vi "DepthProfiling_3D_Core.vi"(5 "BioMAP file path":path=path "", 7 "Params.":variant, 8 "error in (no error)":errorcluster, 9 "Dynamic Params queue":refnum<queue>, 10 "Quit_UserEvent":refnum<user-event>, 11 "ControlQueueRef":variant) -> (0 "error out":errorcluster, 2 "Output":variant)   [LabVIEW 2013]
uses:
  Apps_static/ScanParams_SingleLine.ctl
  ProcessMethods/Binning/BinType.ctl
  Files/BinaryHeader.ctl
  ControlDef/QueueRefs.ctl
  ControlDef/LaserCtrl_Method.ctl
  ControlDef/States-AToF.ctl
  <instrlib>/AnalogDiscSDKLv/VIs/DWF_CtrlQueue.ctl
  <instrlib>/AnalogDiscSDKLv/VIs/DWF_State.ctl
  <instrlib>/ESP300/Public/Data/ESP300_State.ctl
  <instrlib>/DG535/Command/DG535_States.ctl
  Hardware/BNC(QuantumComposers)/BNC_States.ctl
  Hardware/FemtoLaser(Legacy)/Laser_Status.ctl
  Hardware/DAQmx(Legacy)/DAQmx_Status.ctl
  ControlDef/Signal.ctl
  ProcessMethods/SignalAverager/ProcessStates.ctl
  Files/WriterState.ctl
  Files/Signal_Segment.ctl
  ControlDef/ProcessingMode.ctl
  Hardware/EPM2000(Legacy)/EPM2K_Status.ctl
  <instrlib>/AnalogDiscSDKLv/VIs/DWF_Signal.ctl
  ControlDef/SampleRateSelector.ctl
  ImagingMS/DirectImaging_State.ctl
  ImagingMS/Imaging_Params.ctl
  ProcessMethods/BioMapConversion/BioMAPWriterCoreParams.ctl
  <vilib>/Utility/error.llb/DialogType.ctl
  <vilib>/Utility/miscctls.llb/LVRowAndColumnTypeDef.ctl
  <vilib>/picture/picture.llb/imagedata.ctl
  <vilib>/Analysis/baseanly.llb/Mean (DBL).vi
  UI/Autoscale_Y_Single.vi
  <userlib>/_OpenG.lib/comparison/comparison.llb/I32 Changed__ogtk.vi
  ProcessMethods/Binning/SpectrumBinning.vi
  <vilib>/regexp/Match Regular Expression.xnode
  <instrlib>/ESP300/ESP300.lvlib
  <instrlib>/DG535/SRS_DG535_Lib.lvlib
  <userlib>/Utility/ErrorLog_lib.lvlib
  <instrlib>/AnalogDiscSDKLv/AnalogDiscSDKLv.lvlib
  <vilib>/Analysis/NI_AALBase.lvlib
panel:
  out "m/z":dbl=11.0
  in  "Linear/Log":bool
  in  "Integration Width (±Da)":dbl=0.5
  in  "m/z (Da)":dbl=11.0
  in  "BinType":T1=enum."ByMass"
  in  "BinWidth":dbl=0.2 min=0.001
  in  "#Layers":i32=1 caption="LayerAverage#" min=1 max=2000 step=1
  in  "Shot#":i32=1 caption="nth of Shot" min=1 max=65535 step=1
  in  "X--":bool
  in  "X++":bool
  in  "Fullscale X":bool
  in  "Fullscale Y":bool
  in  "Y--":bool
  in  "Y++":bool
  out "Depth Profile":dbl[](graph)
  out "Spectra":cluster{"Array":dbl[], dbl[]}(graph)
  in  "MaxiMass":dbl=300.0 format="%#_13g"
  in  "EnableBinning":bool
  out "Information":string
  in  "AutoScaleZ":bool
  in  "SaveMiddleFile":bool
  in  "Color Scheme":T2(ring)=enum."Rainbow"
  out "#SOL":i32
  out "#EOL":i32
  out "remaining lines":i32
  out "State":T3(ring)
  out "Line#":i32
  in  "Cancel":bool
  in  "Close/Quit":bool
  in  "Peaks of Interest":string[][](table)=[["300", "300"], ["68", ".45"], ["92", ".45"], ["114", ".45"]]
  in  "conv. coeff.":sgl=6553.0
  out "# average":i32
  in  "Start":bool
  out "ImagePreview":dbl[][](graph)
  in  "PeakOI #":i32
  out "MS (Raw)":cluster{"m/z_Array":dbl[], sgl[]}(graph)
  out "Iteration":i32
  out "Export File Path":path caption="Filename"
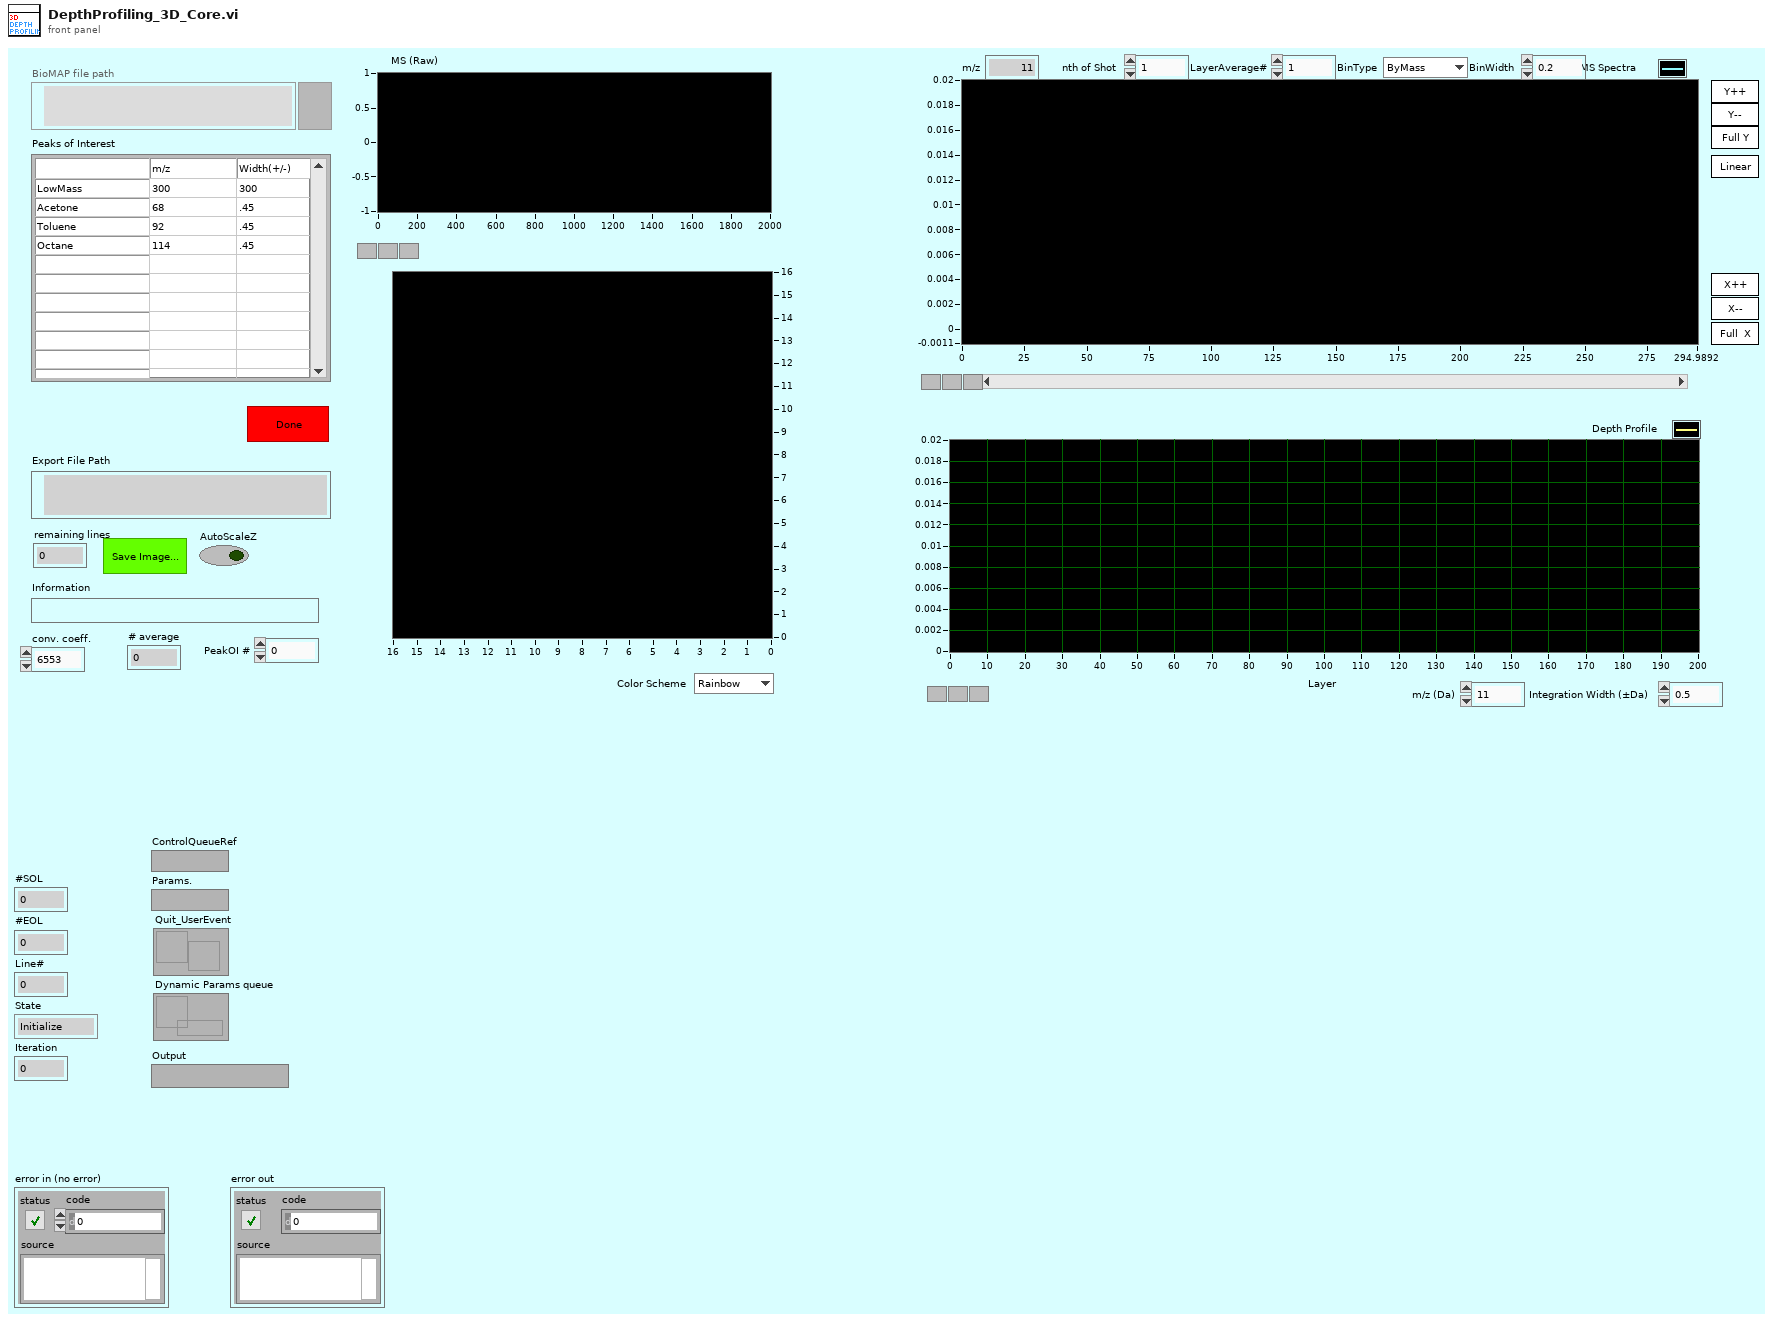
[diagram p1: front panel]
types:
  T1 = typedef "BinType.ctl" = enum16{"ByTime", "ByScreen", "ByMass", "ToUnitMass"}
  T2 = enum16{"Greyscale", "Rainbow", "Jet", "Rainbow_Wh", "Banded", "Seis", "InvertSeis", "Jaisnd", "TBD1"}
  T3 = enum16{"Initialize", "Open", "PrepScanParams", "WaitData", "Flush", "ScanResult", "CheckEndCondition", "Close", "Quit", "Refresh_Image", "Refresh_Profile", "Refresh_Spectra", "Refresh_RawSpectrum", "SaveMiddleFile", "Save_Image", "SetPeakOI"}
  T4 = cluster{"image path":path, "file refnum":refnum<file>}
  T5 = enum8{"Enabled", "Disabled", "Disabled and Grayed Out"}
  T6 = typedef "QueueRefs.ctl" = cluster{"LaserCtrlMethod":T7, "Apps":refnum<queue>, "MainDAQCoreQueue":refnum<queue>, "Micos":refnum<queue>, "ESP300":refnum<queue>, "SMC100":refnum<queue>, "SRS DG535":refnum<queue>, "BNC":refnum<queue>, "SDG_ii":refnum<queue>, "NI-USB_DAQmx":refnum<queue>, "ProcCore_CtrlQueue":refnum<queue>, "WriterCtrl":refnum<queue>, "WriterSIG":refnum<queue>, "Feedback":refnum<queue>, "EPM2000":refnum<queue>, "InfoRef":refnum<vi>, "AppsLock":T8, "ProcCore_SignalQueue":refnum<queue>}
  T7 = typedef "LaserCtrl_Method.ctl" = enum16{"SRS_DG535", "BNC", "SDG_II"}
  T8 = typedef "Semaphore RefNum" = refnum<k1>
  T9 = typedef "ProcessStates.ctl" = enum16{"Initialize", "Normal", "Display", "Write2Buffer", "CalcMzArray", "StartSave", "StopSave", "ConfigChanged", "EndOfLine", "SetFilterParams", "SetGraphsEnable", "SetAcquisitionParams", "ChangeDisplayIncrement", "ChangeRepRate", "SetWriterRef", "Quit", "StartOfLine"}
  T10 = cluster{"Average":i32, "X (Img)":i32, "Y (Img)":i32, "Spectra":sgl[], "Depth":i32, "TickCount":dbl}
  T11 = typedef "BioMAPWriterCoreParams.ctl" = cluster{"File Header":T12, "mzCali.":dbl[], "m/z_Array":dbl[], "SampleRate":T13, "TrigDelay":dbl, "file refnum":refnum<file>, "file path":path, "PeakOI":cluster{"m/z":dbl, "Width(+/-)":dbl}[], "Binning":cluster{"Enable":bool, "BinType":T1, "BinWidth":dbl, "Maximum":dbl, "Minimum":dbl}}
  T12 = typedef "BinaryHeader.ctl" = cluster{"Start Position":dbl[], "StepWidth":dbl[], "Dimension":i32[], "SpecLength":i32}
  T13 = typedef "SampleRateSelector.ctl" = dbl
  T14 = typedef "Imaging_Params.ctl" = cluster{"File Header":T12, "ScanSpeed":dbl, "HighSpeed":dbl, "SampleRate":T13, "Rep.Rate (Hz)":dbl, "TrigDelay":dbl, "mzCali":dbl[], "KeepStill(ms)":u32, "SaveRaw":bool}
  T15 = typedef "DirectImaging_State.ctl" = cluster{"State":enum16{"Initialize", "Open", "PrepScanParams", "WaitData", "Flush", "ScanResult", "CheckEndCondition", "Close", "Quit", "Refresh_Image", "Refresh_Profile", "Refresh_Spectra", "Refresh_RawSpectrum", "SaveMiddleFile", "Save_Image", "SetPeakOI"}, "Para.":variant}
  T16 = cluster{"Save?":bool, "File Header":T12, "Scan#":i32, "ControlRefs":T6, "HighSpeed":dbl, "ScanSpeed":dbl, "SampleRate":T13, "mzCali.":dbl[], "TrigDelay":dbl, "InfoBarRef.":refnum<vi>, "mzArray":dbl[], "SaveRaw":bool, "RepRate":dbl, "Z_Counter":i32}
  T17 = typedef "LVRowAndColumnTypeDef.ctl" = cluster{"Row":i32, "Column":i32}
  T18 = typedef "DialogType.ctl" = u16
  T19 = typedef "LVPoint32TypeDef.ctl" = cluster{"Horizontal":i32, "Vertical":i32}
  T20 = typedef "LVRectTypeDef.ctl" = cluster{"Left":i16, "Top":i16, "Right":i16, "Bottom":i16}
  T21 = enum16{"open", "replace", "create", "open or create", "replace or create", "replace or create with confirmation"}
  T22 = cluster{"queue out":refnum<queue>, "queue out":refnum<queue>}
  T23 = typedef "Signal.ctl" = cluster{"Command":T9, "Params":variant}
  T24 = typedef "Signal_Segment.ctl" = cluster{"SampleRate":dbl, "TrigDelay":dbl, "SpecLength":dbl, "DAQ_Range":dbl, "Average#":i32, "Position":dbl[], "Spectrum":sgl[], "Calibr.":dbl[], "Pressure":dbl, "Desp_LaserEnergy":dbl, "PI_LaserEnergy":dbl, "Voltages Table":sgl[][], "ProcMode":T25, "Threshold":dbl, "Comment":string, "TickCount":dbl, "Time Stamp":timestamp}
  T25 = typedef "ProcessingMode.ctl" = enum16{"None", "Drop by Threshold", "TDC Simulate", "SetFilter"}
  T26 = typedef "ScanParams_SingleLine.ctl" = cluster{"Line Start":dbl[], "Line End":dbl[], "HighSpeed":dbl, "ScanSpeed":dbl, "KeepStill(ms)":u32, "InstruParams":dbl[]}
  T27 = typedef "imagedata.ctl" = cluster{"image type":i32, "image depth":i32, "image":u8[], "mask":u8[], "colors":u32[], "Rectangle":cluster{"left":i16, "top":i16, "right":i16, "bottom":i16}}
  T28 = cluster{"Rows Per Strip":i32, "Photometric":i32, "Compression Type":i32}
  T29 = cluster{"Average":i32, "X (Img)":i32, "Y (Img)":i32, "Spectra":sgl[], "Depth":i32, "TickCount":dbl}[]
  T30 = typedef "IMAQ Image.ctl" = refnum<image>
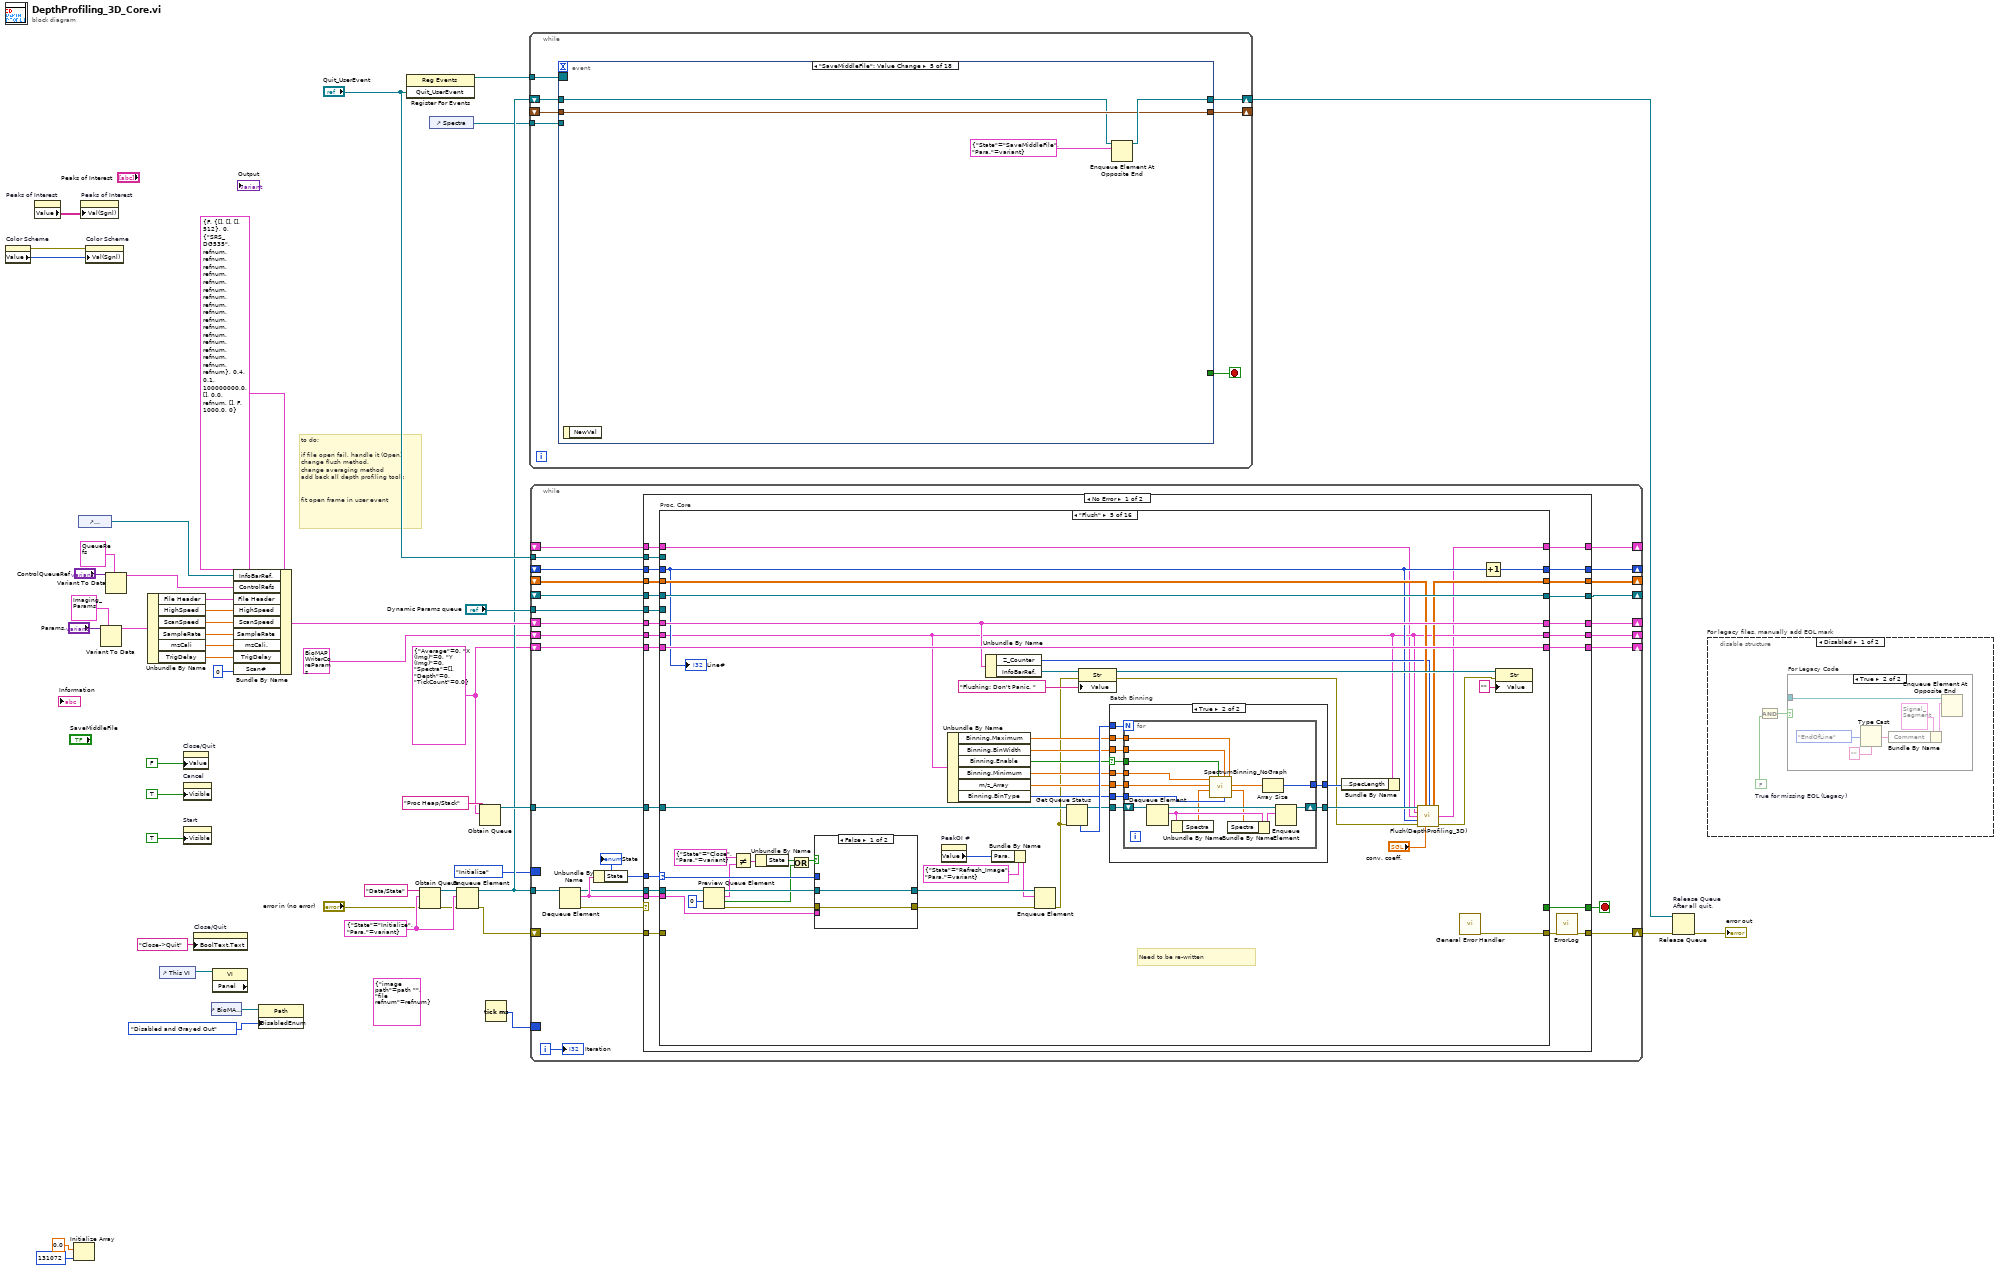
[diagram p0: block diagram]
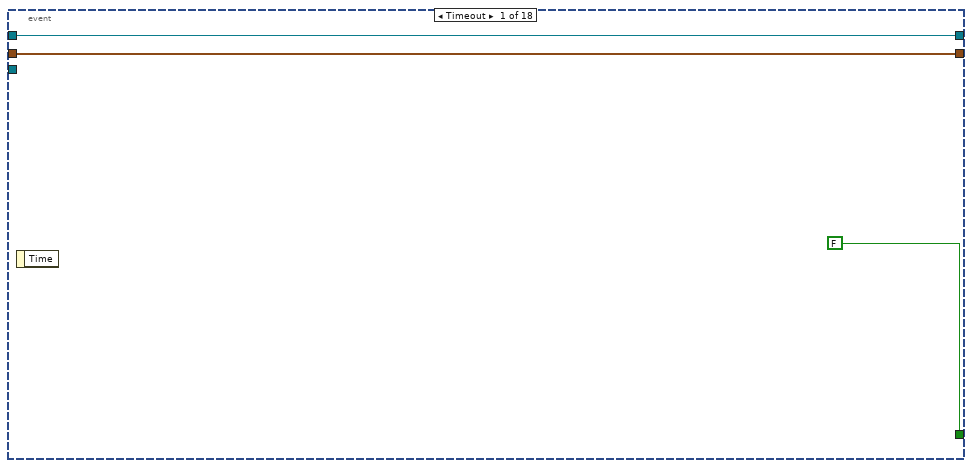
[diagram p4: hidden frame]
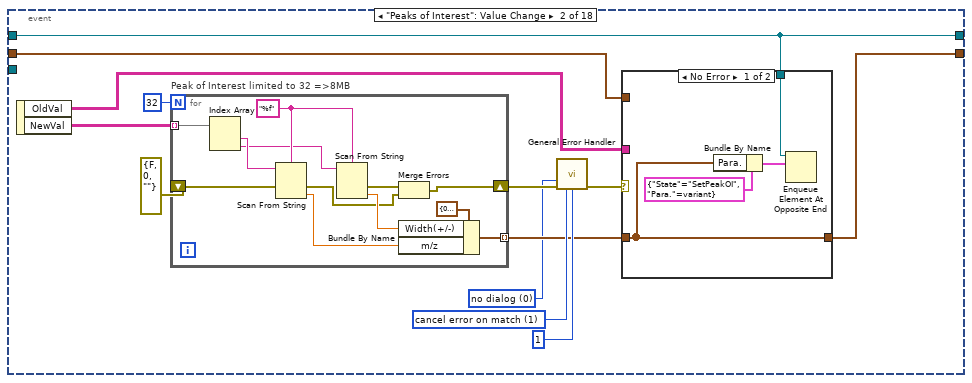
[diagram p5: hidden frame]
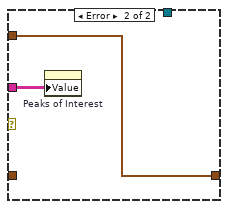
[diagram p6: hidden frame]
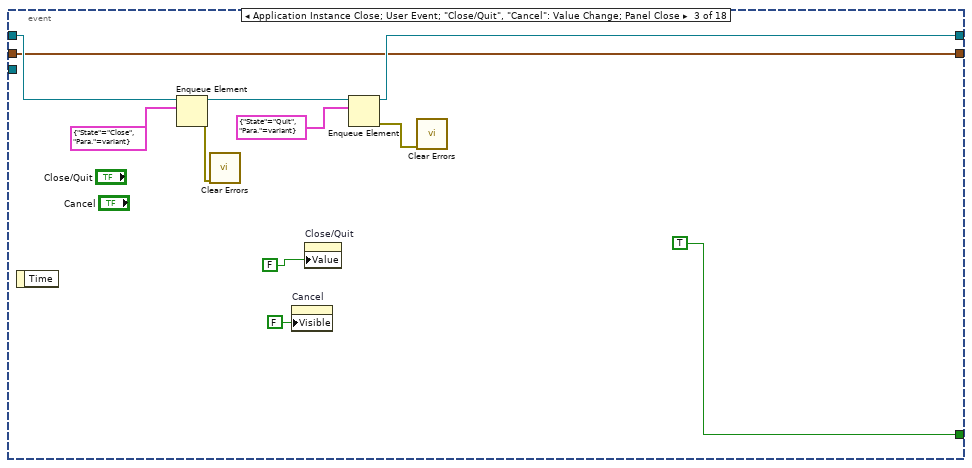
[diagram p7: hidden frame]
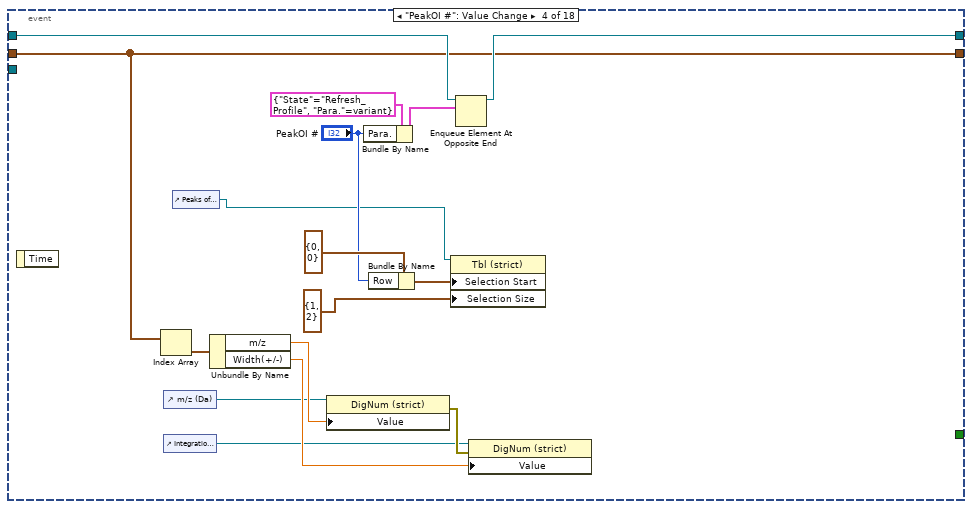
[diagram p8: hidden frame]
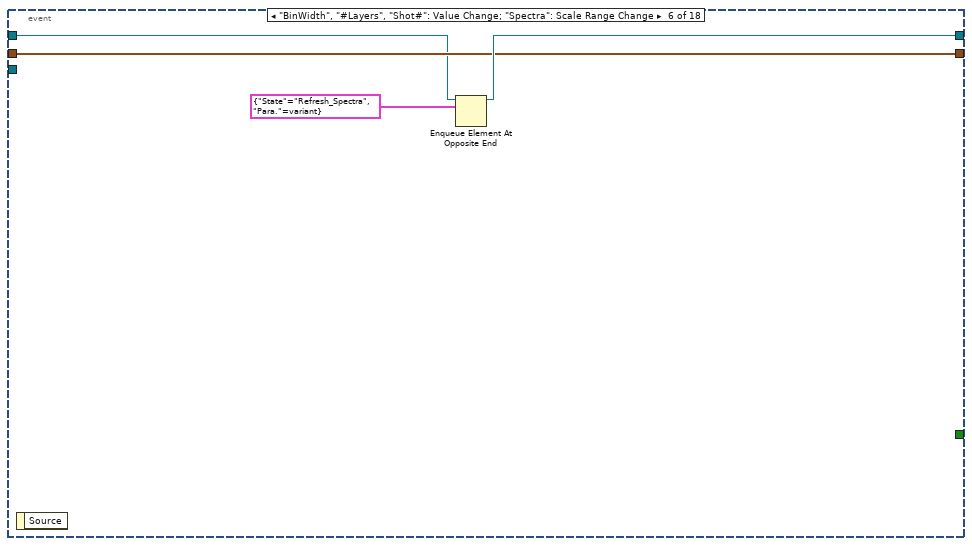
[diagram p9: hidden frame]
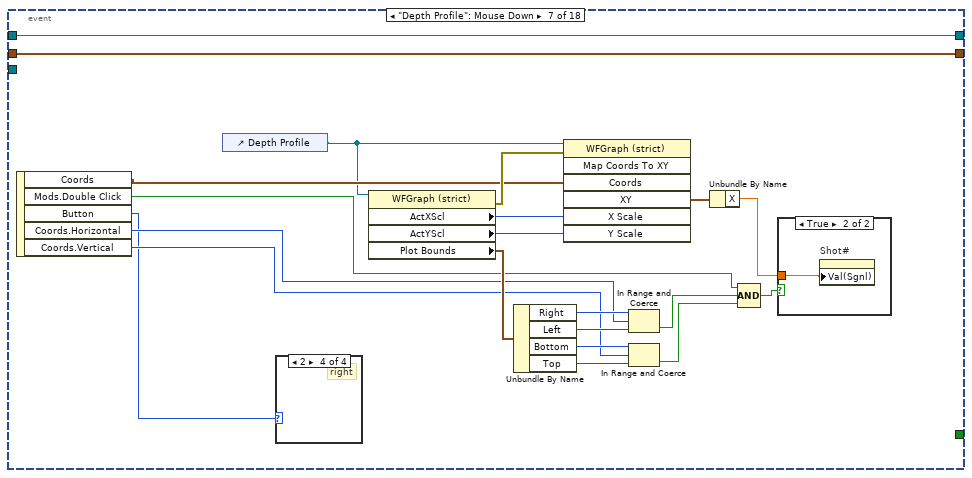
[diagram p10: hidden frame]
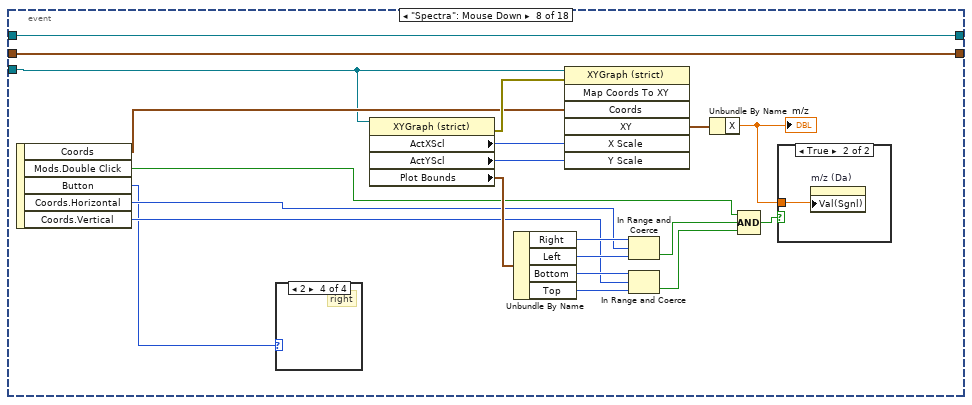
[diagram p15: hidden frame]
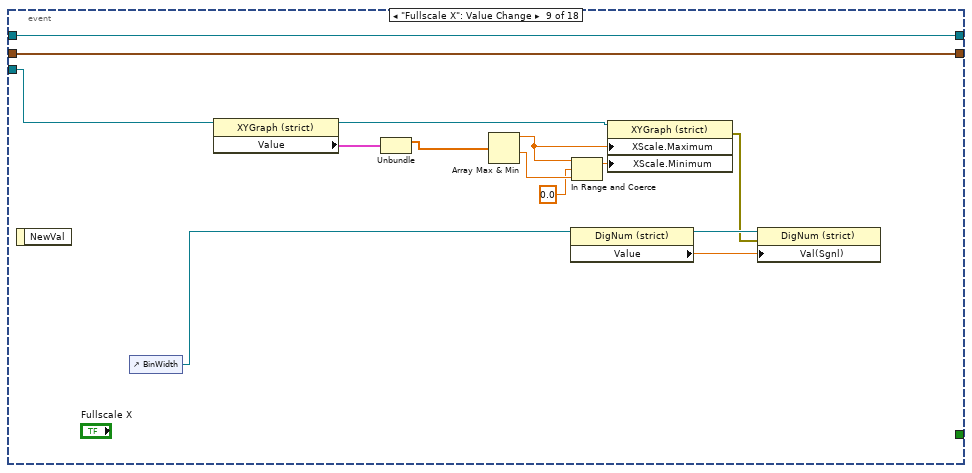
[diagram p20: hidden frame]
diagram:
  (unwired) T4 {"image path"=path "", "file refnum"=refnum} ("output cluster")
  w26 = T10 {"Average"=0, "X (Img)"=0, "Y (Img)"=0, "Spectra"=[], "Depth"=0, "TickCount"=0.0} ("output cluster")
  w38 = T15 {"State"=enum."Initialize", "Para."=variant}
  # "to do;\n\nif file open fail, handle it (Open)\nchange flush method,\nchange averaging method\nadd back all depth profiling tools\n\n\nfit open frame in user event"
  n1 = property on="Color Scheme" class="Enum (strict)"() -> (error out=w2:errorcluster, "Value"=w3:T2)  [unwired: 2 in, 1 out]
  n2 = property on="Peaks of Interest" class="Tbl (strict)"() -> ("Value"=w7:string[][])  [unwired: 2 in, 2 out]
  n3 = Initialize Array(sgl 0.0 ("element"), 131072 ("dimension size")) -> ()  [unwired: 1 out]
  n4 = control-ref of="Information"() -> (w5:refnum<vi>)
  n5 = property on="Peaks of Interest" class="Tbl (strict)"("Val(Sgnl)"=w7) -> ()  [unwired: 2 in, 2 out]
  n6 = property on="Color Scheme" class="Enum (strict)"(error in=w2, "Val(Sgnl)"=w3) -> ()  [unwired: 1 in, 2 out]
  n7 = Variant To Data(type=T14 {"File Header"={"Start Position"=[], "StepWidth"=[], "Dimension"=[], "SpecLength"=0}, "ScanSpeed"=0.0, "HighSpeed"=0.0, "SampleRate"=0.0, "Rep.Rate (Hz)"=0.0, "TrigDelay"=0.0, "mzCali"=[], "KeepStill(ms)"=0, "SaveRaw"=FALSE} ("BeamProfiling_Params"), Variant="Params.") -> (data=w33:T14)  [unwired: 1 in, 1 out]
  n8 = Variant To Data(type=T6 {"LaserCtrlMethod"=enum."SRS_DG535", "Apps"=refnum, "MainDAQCoreQueue"=refnum, "Micos"=refnum, "ESP300"=refnum, "SMC100"=refnum, "SRS DG535"=refnum, "BNC"=refnum, "SDG_ii"=refnum, "NI-USB_DAQmx"=refnum, "ProcCore_CtrlQueue"=refnum, "WriterCtrl"=refnum, "WriterSIG"=refnum, "Feedback"=refnum, "EPM2000"=refnum, "InfoRef"=refnum, "AppsLock"=refnum, "ProcCore_SignalQueue"=refnum} ("ControlRefs"), Variant="ControlQueueRef") -> (data=w13:T6)  [unwired: 1 in, 1 out]
  n9 = Unbundle By Name(w33) -> ("File Header"=w32:T12, "HighSpeed"=w31:dbl, "ScanSpeed"=w30:dbl, "SampleRate"=w28:T13, "mzCali"=w19:dbl[], "TrigDelay"=w18:dbl)
  n10 = control-ref of="This VI"() -> (w17:refnum<vi>)
  n11 = property on="Close/Quit" class="Bool (strict)"("Value"=FALSE) -> ()  [unwired: 2 in, 2 out]
  n12 = property on="Cancel" class="Bool"("Visible"=TRUE) -> ()  [unwired: 2 in, 2 out]
  n13 = property on="Start" class="Bool"("Visible"=TRUE) -> ()  [unwired: 2 in, 2 out]
  n14 = property on="Close/Quit" class="Bool (strict)"("BoolText.Text"="Close->Quit" ("Boolean Text.Text")) -> ()  [unwired: 2 in, 2 out]
  n15 = control-ref of="BioMAP file path"() -> (w12:refnum<vi>)
  n16 = property class="VI" props=["Panel"](reference=w17) -> ()  [unwired: 1 in, 3 out]
  n17 = Bundle By Name(cluster=T16 {"Save?"=FALSE, "File Header"={"Start Position"=[], "StepWidth"=[], "Dimension"=[], "SpecLength"=512}, "Scan#"=0, "ControlRefs"={"LaserCtrlMethod"=enum."SRS_DG535", "Apps"=refnum, "MainDAQCoreQueue"=refnum, "Micos"=refnum, "ESP300"=refnum, "SMC100"=refnum, "SRS DG535"=refnum, "BNC"=refnum, "SDG_ii"=refnum, "NI-USB_DAQmx"=refnum, "ProcCore_CtrlQueue"=refnum, "WriterCtrl"=refnum, "WriterSIG"=refnum, "Feedback"=refnum, "EPM2000"=refnum, "InfoRef"=refnum, "AppsLock"=refnum, "ProcCore_SignalQueue"=refnum}, "HighSpeed"=0.4, "ScanSpeed"=0.1, "SampleRate"=100000000.0, "mzCali."=[], "TrigDelay"=0.0, "InfoBarRef."=refnum, "mzArray"=[], "SaveRaw"=FALSE, "RepRate"=1000.0, "Z_Counter"=0} ("output cluster"), "InfoBarRef."=w5, "ControlRefs"=w13, "File Header"=w32, "HighSpeed"=w31, "ScanSpeed"=w30, "SampleRate"=w28, "mzCali."=w19, "TrigDelay"=w18, "Scan#"=0) -> (w42:T16)
  n18 = property class="Path"(reference=w12, "DisabledEnum"=T5."Disabled and Grayed Out" ("Disabled")) -> ()  [unwired: 1 in, 2 out]
  n19 = register-events("Quit_UserEvent") -> (reference out=w43:refnum<event-registration>)  [unwired: 2 in, 1 out]
  n20 = Obtain Queue(name (unnamed)="Data/State", element data type=w38, error in (no error)="error in (no error)") -> (queue out=w39:refnum<queue>, error out=w37:errorcluster)  [unwired: 2 in, 1 out]
  n21 = control-ref of="Spectra"() -> (w1:refnum<vi>)
  n22 = Enqueue Element(queue=w39, element=w38, error in (no error)=w37) -> (queue out=w35:refnum<queue>, error out=w27:errorcluster)  [unwired: 1 in, 1 out]
  n23 = Obtain Queue(name (unnamed)="Proc Heap/Stack", element data type=w26) -> (queue out=w48:refnum<queue>)  [unwired: 3 in, 2 out]
  n24 = Tick Count (ms)() -> (millisecond timer value=w25:u32)
  n25 = while {
    tunnel: w43 -> [w53]
    shift-right: [w52] -> w20
    shift-left: w35 -> [w55]
    shift-right: [w51] -> _
    shift-left: _ -> [w50]
    tunnel: w1 -> [w49]
    stop <- w54 stop-if-true
    n26 = event shown="[4] \"SaveMiddleFile\": Value Change" {
      selector: w53 -> [_ _ _ _ _ _ _ _ _ _ _ _ _ _ _ _ _ _]
      dyn-events: _ -> [_ _ _ _ _ _ _ _ _ _ _ _ _ _ _ _ _ _]
      timeout: _ -> [_ _ _ _ _ _ _ _ _ _ _ _ _ _ _ _ _ _]
      tunnel: w55 -> [w57 w59 w97 w113 w117 w121 w145 w167 w182 w185 w192 w210 w228 w250 w279 w290 w313 w345]
      tunnel: [FALSE _ TRUE _ _ _ _ _ _ _ _ _ _ _ _ _ _ _] -> w54
      tunnel: [w57 w59 w93 w114 w119 w123 w145 w167 w182 w185 w192 w210 w228 w250 w279 w290 w308 w344] -> w52
      tunnel: [w56 w64 w92 w104 w118 w122 w144 w166 w181 w184 w191 w209 w227 w249 w278 w287 w310 w343] -> w51
      tunnel: w50 -> [w56 w62 w92 w104 w118 w122 w144 w166 w181 w184 w191 w209 w227 w249 w278 w287 w310 w343]
      tunnel: w49 -> [_ _ _ _ _ _ _ w147 w169 w183 w187 w193 w211 w229 w258 _ _ _]
      event Timeout {
        n27 = event-data() -> ()  [unwired: 1 in, 1 out]
      }
      event "Peaks of Interest": Value Change {
        w60 = T18 0 items=["no dialog", "OK message", "continue or stop message", "OK message + warnings", "continue/stop + warnings"] ("type of dialog (OK msg:1)")
        w65 = 1 items=["no exception", "cancel error on match", "set error on match"] ("[exception action] (none:0)")
        n28 = event-data() -> ("OldVal"=w70:string[][], "NewVal"=w71:string[][])  [unwired: 1 in]
        n29 = for "Peak of Interest limited to 32 =>8MB" {
          N: 32 -> [_]
          tunnel: w71 -> [w83] mode=indexing
          shift-right: [w75] -> w66
          shift-left: errorcluster {"status"=FALSE, "code"=0, "source"=""} ("error IO") -> [w77]
          tunnel: [w76] -> w63 mode=indexing
          w82 = "%f" ("format string")
          n30 = Index Array(array=w83) -> (element #1=w73:string, element #2=w72:string)  [unwired: 2 in]
          n31 = Scan From String(format string=w82, input string=w73, error in=w77) -> (error out=w74:errorcluster, output 1=w79:dbl)  [unwired: 2 in, 2 out]
          n32 = Scan From String(format string=w82, input string=w72) -> (error out=w78:errorcluster, output 1=w80:dbl)  [unwired: 3 in, 2 out]
          n33 = Merge Errors(w78, w74) -> (w75:errorcluster)
          n34 = Bundle By Name(cluster=cluster{"m/z":dbl, "Width(+/-)":dbl} {"m/z"=0.0, "Width(+/-)"=0.0} ("Peak-Of-Interest"), "Width(+/-)"=w80, "m/z"=w79) -> (w76:cluster{"m/z":dbl, "Width(+/-)":dbl})
        }
        n35 = call <vilib>:"General Error Handler.vi"("type of dialog (OK msg:1)"=w60, "error in (no error)"=w66, "[exception action] (none:0)"=w65, "[exception code]"=1) -> ("error out"=w67:errorcluster)  [unwired: 7 in, 4 out]
        n36 = case shown="No Error" w67 {
          tunnel: w70 -> [_ w89]
          tunnel: [w85 w88] -> w64
          tunnel: w63 -> [w85 _]
          tunnel: w62 -> [_ w88]
          tunnel: w59 -> [w84 _]
          frame No Error {
            n37 = Bundle By Name(cluster=T15 {"State"=enum."SetPeakOI", "Para."=variant} ("element"), "Para."=w85) -> (w86:T15)
            n38 = Enqueue Element At Opposite End(queue=w84, element=w86) -> ()  [unwired: 2 in, 3 out]
          }
          frame Error {
            n39 = property on="Peaks of Interest" class="Tbl (strict)"("Value"=w89) -> ()  [unwired: 2 in, 2 out]
          }
        }
      }
      event Application Instance Close; User Event; "Close/Quit", "Cancel": Value Change; Panel Close {
        n40 = event-data() -> ()  [unwired: 1 in, 1 out]
        n41 = Enqueue Element(queue=w97, element=T15 {"State"=enum."Close", "Para."=variant}) -> (queue out=w98:refnum<queue>, error out=w96:errorcluster)  [unwired: 2 in, 1 out]
        n42 = call <vilib>:"Clear Errors.vi"("error in (no error)"=w96) -> ()  [unwired: 6 in, 1 out]
        n43 = property on="Cancel" class="Bool"("Visible"=FALSE) -> ()  [unwired: 2 in, 2 out]
        n44 = property on="Close/Quit" class="Bool (strict)"("Value"=FALSE) -> ()  [unwired: 2 in, 2 out]
        n45 = Enqueue Element(queue=w98, element=T15 {"State"=enum."Quit", "Para."=variant}) -> (queue out=w93:refnum<queue>, error out=w99:errorcluster)  [unwired: 2 in, 1 out]
        n46 = call <vilib>:"Clear Errors.vi"("error in (no error)"=w99) -> ()  [unwired: 6 in, 1 out]
      }
      event "PeakOI #": Value Change {
        n47 = event-data() -> ()  [unwired: 1 in, 1 out]
        n48 = Index Array(array=w104) -> (element=w105:cluster{"m/z":dbl, "Width(+/-)":dbl})  [unwired: 1 in]
        n49 = control-ref of="m/z (Da)"() -> (w102:refnum<vi>)
        n50 = control-ref of="Integration Width (±Da)"() -> (w101:refnum<vi>)
        n51 = control-ref of="Peaks of Interest"() -> (w108:refnum<vi>)
        n52 = Unbundle By Name(w105) -> ("m/z"=w103:dbl, "Width(+/-)"=w106:dbl)
        n53 = property class="DigNum (strict)"(reference=w102, "Value"=w103) -> (error out=w107:errorcluster)  [unwired: 1 in, 1 out]
        n54 = Bundle By Name(cluster=T15 {"State"=enum."Refresh_Profile", "Para."=variant} ("element"), "Para."="PeakOI #") -> (w115:T15)
        n55 = Bundle By Name(cluster=T17 {"Row"=0, "Column"=0} ("Selection Start"), "Row"="PeakOI #") -> (w111:T17)
        n56 = property on="Property Node" class="Tbl (strict)"(reference=w108, "Selection Start"=w111, "Selection Size"=T17 {"Row"=1, "Column"=2}) -> ()  [unwired: 1 in, 2 out]
        n57 = Enqueue Element At Opposite End(queue=w113, element=w115) -> (queue out=w114:refnum<queue>)  [unwired: 2 in, 2 out]
        n58 = property class="DigNum (strict)"(reference=w101, error in=w107, "Value"=w106) -> ()  [unwired: 2 out]
      }
      event "SaveMiddleFile": Value Change {
        n59 = event-data() -> ()  [unwired: 1 in, 1 out]
        n60 = Enqueue Element At Opposite End(queue=w117, element=T15 {"State"=enum."SaveMiddleFile", "Para."=variant}) -> (queue out=w119:refnum<queue>)  [unwired: 2 in, 2 out]
      }
      event "BinWidth", "#Layers", "Shot#": Value Change; "Spectra": Scale Range Change {
        n61 = event-data() -> ()  [unwired: 1 in, 1 out]
        n62 = Enqueue Element At Opposite End(queue=w121, element=T15 {"State"=enum."Refresh_Spectra", "Para."=variant}) -> (queue out=w123:refnum<queue>)  [unwired: 2 in, 2 out]
      }
      event "Depth Profile": Mouse Down {
        n63 = event-data() -> ("Coords"=w126:T19, "Mods.Double Click"=w127:bool, "Button"=w128:u16, "Coords.Horizontal"=w129:i32, "Coords.Vertical"=w130:i32)  [unwired: 1 in]
        n64 = control-ref of="Depth Profile"() -> (w125:refnum<vi>)
        n65 = case shown="2" w128 {
          frame Default {
          }
          frame 3 {
            # "middle"
          }
          frame 1 {
            # "left"
          }
          frame 2 {
            # "right"
          }
        }
        n66 = property on="Property Node" class="WFGraph (strict)"(reference=w125) -> (error out=w131:errorcluster, "ActXScl"=w134:i32, "ActYScl"=w133:i32, "Plot Bounds"=w136:T20)  [unwired: 1 in, 1 out]
        n67 = Unbundle By Name(w136) -> ("Right"=w137:i16, "Left"=w138:i16, "Bottom"=w139:i16, "Top"=w140:i16)
        n68 = invoke on="Invoke Node" class="WFGraph (strict)" method="Map Coords To XY"(reference=w125, error in=w131, "Coords"=w126, "X Scale"=w134, "Y Scale"=w133) -> ("XY"=w132:cluster{"X":dbl, "Y":dbl})  [unwired: 2 in, 6 out]
        n69 = In Range and Coerce(upper limit=w137, x=w129, lower limit=w138) -> (In Range?=w142:bool)  [unwired: 1 out]
        n70 = In Range and Coerce(upper limit=w139, x=w130, lower limit=w140) -> (In Range?=w143:bool)  [unwired: 1 out]
        n71 = Unbundle By Name(w132) -> ("X"=w135:dbl)
        n72 = Compound Arithmetic op=AND(w127, w142, w143) -> (w141:bool)
        n73 = case shown="True" w141 {
          tunnel: w135 -> [_ w146]
          frame False {
          }
          frame True {
            n74 = property on="Shot#" class="DigNum (strict)"("Val(Sgnl)"=w146) -> ()  [unwired: 2 in, 2 out]
          }
        }
      }
      event "Spectra": Mouse Down {
        n75 = event-data() -> ("Coords"=w149:T19, "Mods.Double Click"=w150:bool, "Button"=w151:u16, "Coords.Horizontal"=w152:i32, "Coords.Vertical"=w153:i32)  [unwired: 1 in]
        n76 = case shown="2" w151 {
          frame Default {
          }
          frame 3 {
            # "middle"
          }
          frame 1 {
            # "left"
          }
          frame 2 {
            # "right"
          }
        }
        n77 = property on="Property Node" class="XYGraph (strict)"(reference=w147) -> (error out=w154:errorcluster, "ActXScl"=w157:i32, "ActYScl"=w156:i32, "Plot Bounds"=w158:T20)  [unwired: 1 in, 1 out]
        n78 = Unbundle By Name(w158) -> ("Right"=w159:i16, "Left"=w160:i16, "Bottom"=w161:i16, "Top"=w162:i16)
        n79 = invoke on="Invoke Node" class="XYGraph (strict)" method="Map Coords To XY"(reference=w147, error in=w154, "Coords"=w149, "X Scale"=w157, "Y Scale"=w156) -> ("XY"=w155:cluster{"X":dbl, "Y":dbl})  [unwired: 2 in, 6 out]
        n80 = In Range and Coerce(upper limit=w159, x=w152, lower limit=w160) -> (In Range?=w164:bool)  [unwired: 1 out]
        n81 = In Range and Coerce(upper limit=w161, x=w153, lower limit=w162) -> (In Range?=w165:bool)  [unwired: 1 out]
        n82 = Unbundle By Name(w155) -> ("X"=w148:dbl)
        "m/z" <- w148
        n83 = Compound Arithmetic op=AND(w150, w164, w165) -> (w163:bool)
        n84 = case shown="True" w163 {
          tunnel: w148 -> [_ w168]
          frame False {
          }
          frame True {
            n85 = property on="m/z (Da)" class="DigNum (strict)"("Val(Sgnl)"=w168) -> ()  [unwired: 2 in, 2 out]
          }
        }
      }
      event "Fullscale X": Value Change {
        n86 = event-data() -> ()  [unwired: 1 in, 1 out]
        n87 = control-ref of="BinWidth"() -> (w170:refnum<vi>)
        n88 = property class="XYGraph (strict)"(reference=w169) -> (reference out=w174:refnum<vi>, "Value"=w177:cluster{"Array":dbl[], dbl[]})  [unwired: 1 in, 1 out]
        n89 = Unbundle(w177) -> ("Array"=w176:dbl[])  [unwired: 1 out]
        n90 = Array Max & Min(array=w176) -> (max value=w175:dbl, min value=w180:dbl)  [unwired: 2 out]
        n91 = property class="DigNum (strict)"(reference=w170) -> (reference out=w173:refnum<vi>, "Value"=w172:dbl)  [unwired: 1 in, 1 out]
        n92 = In Range and Coerce(upper limit=w175, x=0.0 ("X Scale.Range:Minimum"), lower limit=w180) -> (coerced(x)=w178:dbl)  [unwired: 1 out]
        n93 = property on="Property Node" class="XYGraph (strict)"(reference=w174, "XScale.Maximum"=w175, "XScale.Minimum"=w178) -> (error out=w171:errorcluster)  [unwired: 1 in, 1 out]
        n94 = property class="DigNum (strict)"(reference=w173, error in=w171, "Val(Sgnl)"=w172) -> ()  [unwired: 2 out]
      }
      event "Fullscale Y": Value Change {
        n95 = event-data() -> ()  [unwired: 1 in, 1 out]
        n96 = call-poly "Autoscale_Y.vi"("GraphRef"=w183) -> ()  [unwired: 11 in]
      }
      event "Linear/Log": Value Change {
        n97 = event-data() -> ()  [unwired: 1 in, 6 out]
        n98 = Select(t=u8 1 ("Y Scale.Mapping Mode"), s="Linear/Log", f=u8 0 ("Y Scale.Mapping Mode")) -> (s? t:f=w190:u8)
        n99 = property on="Property Node" class="XYGraph (strict)"(reference=w187, "YScale.Mapping Mode"=w190) -> ()  [unwired: 1 in, 2 out]
      }
      event "X++": Value Change {
        n100 = event-data() -> ()  [unwired: 1 in, 6 out]
        n101 = property on="Property Node" class="XYGraph (strict)"(reference=w193) -> (reference out=w198:refnum<vi>, "XScale.Maximum"=w199:dbl, "XScale.Minimum"=w200:dbl)  [unwired: 1 in, 1 out]
        n102 = Add(x=w199, y=w200) -> (x+y=w201:dbl)
        n103 = Subtract(x=w199, y=w200) -> (x-y=w204:dbl)
        n104 = control-ref of="BinWidth"() -> (w194:refnum<vi>)
        n105 = Multiply(x=0.5, y=w201) -> (x*y=w205:dbl)
        n106 = Multiply(x=0.25, y=w204) -> (x*y=w206:dbl)
        n107 = Add(x=w205, y=w206) -> (x+y=w207:dbl)
        n108 = Subtract(x=w205, y=w206) -> (x-y=w208:dbl)
        n109 = property class="DigNum (strict)"(reference=w194) -> (reference out=w197:refnum<vi>, "Value"=w196:dbl)  [unwired: 1 in, 1 out]
        n110 = property on="Property Node" class="XYGraph (strict)"(reference=w198, "XScale.Maximum"=w207, "XScale.Minimum"=w208) -> (error out=w195:errorcluster)  [unwired: 1 in, 1 out]
        n111 = property class="DigNum (strict)"(reference=w197, error in=w195, "Val(Sgnl)"=w196) -> ()  [unwired: 2 out]
      }
      event "X--": Value Change {
        n112 = event-data() -> ()  [unwired: 1 in, 6 out]
        n113 = property on="Property Node" class="XYGraph (strict)"(reference=w211) -> (reference out=w216:refnum<vi>, "XScale.Maximum"=w217:dbl, "XScale.Minimum"=w218:dbl)  [unwired: 1 in, 1 out]
        n114 = Add(x=w217, y=w218) -> (x+y=w219:dbl)
        n115 = Subtract(x=w217, y=w218) -> (x-y=w222:dbl)
        n116 = control-ref of="BinWidth"() -> (w212:refnum<vi>)
        n117 = Multiply(x=0.5, y=w219) -> (x*y=w223:dbl)
        n118 = Multiply(x=1.0, y=w222) -> (x*y=w224:dbl)
        n119 = Add(x=w223, y=w224) -> (x+y=w225:dbl)
        n120 = Subtract(x=w223, y=w224) -> (x-y=w226:dbl)
        n121 = property class="DigNum (strict)"(reference=w212) -> (reference out=w215:refnum<vi>, "Value"=w214:dbl)  [unwired: 1 in, 1 out]
        n122 = property on="Property Node" class="XYGraph (strict)"(reference=w216, "XScale.Maximum"=w225, "XScale.Minimum"=w226) -> (error out=w213:errorcluster)  [unwired: 1 in, 1 out]
        n123 = property class="DigNum (strict)"(reference=w215, error in=w213, "Val(Sgnl)"=w214) -> ()  [unwired: 2 out]
      }
      event "Y--": Value Change {
        n124 = event-data() -> ()  [unwired: 1 in, 6 out]
        n125 = property on="Property Node" class="XYGraph (strict)"(reference=w229) -> (reference out=w230:refnum<vi>, "Value"=w231:cluster{"Array":dbl[], dbl[]}, "XScale.Maximum"=w243:dbl, "XScale.Minimum"=w242:dbl, "YScale.Maximum"=w234:dbl, "YScale.Minimum"=w233:dbl)  [unwired: 1 in, 1 out]
        n126 = Unbundle(w231) -> ("Array"=w245:dbl[], w244:dbl[])
        n127 = for {
          tunnel: w244 -> [w252] mode=indexing
          tunnel: w245 -> [w256] mode=indexing
          tunnel: w242 -> [w255]
          tunnel: w243 -> [w254]
          tunnel: [w251] -> w241 mode=indexing
          n128 = In Range and Coerce(upper limit=w254, x=w256, lower limit=w255) -> (In Range?=w253:bool)  [unwired: 1 out]
          n129 = case shown="True" w253 {
            tunnel: w252 -> [_ w257]
            tunnel: [_ w257] -> w251
            frame False {
              (unwired) nan
            }
            frame True {
            }
          }
        }
        n130 = Array Max & Min(array=w241) -> (min value=w235:dbl)  [unwired: 3 out]
        n131 = In Range and Coerce(upper limit=w234, x=w235, lower limit=w233) -> (coerced(x)=w232:dbl)  [unwired: 1 out]
        n132 = Subtract(x=w234, y=w232) -> (x-y=w240:dbl)
        n133 = Subtract(x=w232, y=w233) -> (x-y=w238:dbl)
        n134 = Multiply(x=2.0, y=w240) -> (x*y=w247:dbl)
        n135 = Multiply(x=2.0, y=w238) -> (x*y=w237:dbl)
        n136 = Add(x=w232, y=w247) -> (x+y=w246:dbl)
        n137 = Subtract(x=w232, y=w237) -> (x-y=w236:dbl)
        n138 = property on="Property Node" class="XYGraph (strict)"(reference=w230, "YScale.Maximum"=w246, "YScale.Minimum"=w236) -> ()  [unwired: 1 in, 2 out]
      }
      event "Y++": Value Change {
        n139 = event-data() -> ()  [unwired: 1 in, 6 out]
        n140 = property on="Property Node" class="XYGraph (strict)"(reference=w258) -> (reference out=w259:refnum<vi>, "Value"=w260:cluster{"Array":dbl[], dbl[]}, "XScale.Maximum"=w272:dbl, "XScale.Minimum"=w271:dbl, "YScale.Maximum"=w263:dbl, "YScale.Minimum"=w262:dbl)  [unwired: 1 in, 1 out]
        n141 = Unbundle(w260) -> ("Array"=w274:dbl[], w273:dbl[])
        n142 = for {
          tunnel: w273 -> [w281] mode=indexing
          tunnel: w274 -> [w285] mode=indexing
          tunnel: w271 -> [w284]
          tunnel: w272 -> [w283]
          tunnel: [w280] -> w270 mode=indexing
          n143 = In Range and Coerce(upper limit=w283, x=w285, lower limit=w284) -> (In Range?=w282:bool)  [unwired: 1 out]
          n144 = case shown="True" w282 {
            tunnel: w281 -> [_ w286]
            tunnel: [_ w286] -> w280
            frame False {
              (unwired) nan
            }
            frame True {
            }
          }
        }
        n145 = Array Max & Min(array=w270) -> (min value=w264:dbl)  [unwired: 3 out]
        n146 = In Range and Coerce(upper limit=w263, x=w264, lower limit=w262) -> (coerced(x)=w261:dbl)  [unwired: 1 out]
        n147 = Subtract(x=w263, y=w261) -> (x-y=w269:dbl)
        n148 = Subtract(x=w261, y=w262) -> (x-y=w267:dbl)
        n149 = Multiply(x=0.5, y=w269) -> (x*y=w276:dbl)
        n150 = Multiply(x=0.5, y=w267) -> (x*y=w266:dbl)
        n151 = Add(x=w261, y=w276) -> (x+y=w275:dbl)
        n152 = Subtract(x=w261, y=w266) -> (x-y=w265:dbl)
        n153 = property on="Property Node" class="XYGraph (strict)"(reference=w259, "YScale.Maximum"=w275, "YScale.Minimum"=w265) -> ()  [unwired: 1 in, 2 out]
      }
      event "Color Scheme": Value Change {
        n154 = event-data() -> ()  [unwired: 1 in, 6 out]
        n155 = case shown="\"Rainbow_Wh\"" "Color Scheme" {
          tunnel: [u32[] [0, 65793, 131586, 197379, 263172, 328965, 394758, 460551, 526344, 592137, 657930, 723723, 789516, 855309, 921102, 986895, 1052688, 1118481, 1184274, 1250067, 1315860, 1381653, 1447446, 1513239, 1579032, 1644825, 1710618, 1776411, 1842204, 1907997, 1973790, 2039583, 2105376, 2171169, 2236962, 2302755, 2368548, 2434341, 2500134, 2565927, 2631720, 2697513, 2763306, 2829099, 2894892, 2960685, 3026478, 3092271, 3158064, 3223857, 3289650, 3355443, 3421236, 3487029, 3552822, 3618615, 3684408, 3750201, 3815994, 3881787, 3947580, 4013373, 4079166, 4144959, 4210752, 4276545, 4342338, 4408131, 4473924, 4539717, 4605510, 4671303, 4737096, 4802889, 4868682, 4934475, 5000268, 5066061, 5131854, 5197647, 5263440, 5329233, 5395026, 5460819, 5526612, 5592405, 5658198, 5723991, 5789784, 5855577, 5921370, 5987163, 6052956, 6118749, 6184542, 6250335, 6316128, 6381921, 6447714, 6513507, 6579300, 6645093, 6710886, 6776679, 6842472, 6908265, 6974058, 7039851, 7105644, 7171437, 7237230, 7303023, 7368816, 7434609, 7500402, 7566195, 7631988, 7697781, 7763574, 7829367, 7895160, 7960953, 8026746, 8092539, 8158332, 8224125, 8289918, 8355711, 8421504, 8487297, 8553090, 8618883, 8684676, 8750469, 8816262, 8882055, 8947848, 9013641, 9079434, 9145227, 9211020, 9276813, 9342606, 9408399, 9474192, 9539985, 9605778, 9671571, 9737364, 9803157, 9868950, 9934743, 10000536, 10066329, 10132122, 10197915, 10263708, 10329501, 10395294, 10461087, 10526880, 10592673, 10658466, 10724259, 10790052, 10855845, 10921638, 10987431, 11053224, 11119017, 11184810, 11250603, 11316396, 11382189, 11447982, 11513775, 11579568, 11645361, 11711154, 11776947, 11842740, 11908533, 11974326, 12040119, 12105912, 12171705, 12237498, 12303291, 12369084, 12434877, 12500670, 12566463, 12632256, 12698049, 12763842, 12829635, 12895428, 12961221, 13027014, 13092807, 13158600, 13224393, 13290186, 13355979, 13421772, 13487565, 13553358, 13619151, 13684944, 13750737, 13816530, 13882323, 13948116, 14013909, 14079702, 14145495, 14211288, 14277081, 14342874, 14408667, 14474460, 14540253, 14606046, 14671839, 14737632, 14803425, 14869218, 14935011, 15000804, 15066597, 15132390, 15198183, 15263976, 15329769, 15395562, 15461355, 15527148, 15592941, 15658734, 15724527, 15790320, 15856113, 15921906, 15987699, 16053492, 16119285, 16185078, 16250871, 16316664, 16382457, 16448250, 16514043, 16579836, 16645629, 16711422, 16777215] ("Array") w292 w293 w294 w295 w296 w297 w298 u32[] [0, 262147, 589831, 851978, 1179662, 1441811, 1769495, 2031644, 2359328, 2621478, 2949163, 3276848, 3801147, 4194372, 4456520, 4522061, 4718673, 4849750, 5046363, 5177439, 5242980, 5374056, 5439597, 5505142, 5636218, 5767300, 5636232, 5701773, 5701777, 5701782, 5570714, 5505183, 5505187, 5505192, 5177521, 5111990, 5046458, 4980927, 4587720, 4456652, 4325585, 3932374, 3801306, 3604703, 3014888, 2818284, 2621681, 2359541, 2162938, 1638655, 1048831, 786687, 262399, 255, 1279, 4351, 5631, 6655, 7679, 9983, 11007, 12031, 13311, 16383, 17407, 18687, 21759, 23039, 24063, 25087, 27391, 28415, 29439, 30719, 32767, 34815, 36095, 39167, 40447, 41471, 42495, 44799, 45823, 46847, 48127, 50175, 51199, 55551, 56575, 57855, 58879, 59903, 62207, 63231, 64255, 65535, 65526, 65522, 65518, 65505, 65496, 65492, 65483, 65479, 65475, 65471, 65467, 65458, 65454, 65450, 65437, 65432, 65424, 65415, 65411, 65407, 65403, 65394, 65390, 65386, 65382, 65369, 65364, 65360, 65356, 65343, 65339, 65335, 65326, 65322, 65318, 65305, 65301, 65296, 65292, 65288, 65280, 589568, 851712, 1441536, 1703680, 1965824, 2817792, 3079936, 3407616, 3669760, 4194048, 4456192, 4783872, 5046016, 5897984, 6160128, 6422272, 7274240, 7536384, 7864064, 8126208, 8650496, 8912640, 9240320, 9502464, 10092288, 10616576, 10878720, 11730688, 11992832, 12320512, 12582656, 13106944, 13369088, 13696768, 13958912, 14548736, 14810880, 15924992, 16187136, 16449280, 16776960, 16775680, 16773632, 16772608, 16771328, 16770304, 16768256, 16766976, 16765952, 16762624, 16760576, 16759552, 16757248, 16756224, 16755200, 16753920, 16752896, 16750848, 16749568, 16748544, 16745216, 16744192, 16742144, 16739840, 16738816, 16737792, 16736512, 16734464, 16733440, 16732160, 16731136, 16727808, 16726784, 16725760, 16724736, 16721408, 16720384, 16719104, 16717056, 16716032, 16714752, 16711680, 16711680, 16711680, 16711680, 16711680, 16711680, 16711680, 16711680, 16711680, 16711680, 16711680, 16711680, 16711680, 16711680, 16711680, 16711680, 16711680, 16711680, 15527148, 15592941, 15658734, 15724527, 15790320, 15856113, 15921906, 15987699, 16053492, 16119285, 16185078, 16250871, 16316664, 16382457, 16448250, 16514043, 16579836, 16645629, 16711422, 16777215] ("appended array")] -> w288
          frame "Greyscale", Default {
          }
          frame "Rainbow" {
            w292 = u32[] [0, 0, 12517567, 12320960, 12189888, 12058817, 11927746, 11731139, 11600067, 9175197, 9044125, 11141318, 11010246, 10813639, 10682568, 10551497, 10354890, 10223818, 10092747, 7930019, 7798948, 9633997, 9502926, 9306319, 9175248, 9044176, 8847569, 8716498, 8585427, 6750377, 6619306, 8126677, 7995606, 7798999, 7667927, 7536856, 7340249, 7209178, 7078106, 5505199, 5374128, 6619357, 6488285, 6291678, 6160607, 6029536, 5832929, 5701857, 5570786, 4325557, 4194486, 5112036, 4980965, 4784358, 4653287, 4522215, 4325608, 4194537, 4063466, 3080380, 3014844, 3604716, 3408109, 3277038, 3277038, 3145966, 3014895, 2818288, 2687217, 2556145, 1900738, 1769666, 2097396, 1900789, 1769717, 1638646, 1507575, 1310968, 1179896, 1048825, 721096, 590024, 590075, 393468, 262397, 131326, 255, 1791, 3327, 4863, 5068, 6348, 9471, 11007, 12543, 14079, 15615, 17151, 18687, 20223, 17612, 18636, 25087, 26623, 28159, 29695, 31231, 32767, 34303, 35839, 29900, 31180, 40447, 41983, 43775, 45311, 46847, 48383, 49919, 51455, 42444, 43724, 56063, 57599, 59135, 60671, 62207, 63743, 65535, 65528, 52418, 52413, 65510, 65504, 65498, 65492, 65486, 65480, 65474, 65468, 52369, 52364, 65449, 65443, 65437, 65431, 65425, 65419, 65413, 65407, 52321, 52316, 65389, 65383, 65377, 65371, 65364, 65358, 65352, 65346, 52272, 52267, 65328, 65322, 65316, 65310, 65304, 65298, 65292, 65286, 52224, 314368, 851712, 1244928, 1638144, 2031360, 2424576, 2817792, 3211008, 3604224, 3197952, 3525632, 4783872, 5177088, 5635840, 6029056, 6422272, 6815488, 7208704, 7601920, 6409216, 6736896, 6736896, 8781568, 9174784, 9568000, 9961216, 10354432, 10747648, 11206400, 11599616, 9554944, 9882624, 12779264, 13172480, 13565696, 13958912, 14352128, 14745344, 15138560, 15531776, 12766208, 13093888, 16776960, 16775170, 16773637, 16771847, 16770314, 16768780, 16766991, 16765457, 13411088, 13409810, 16760601, 16758812, 16757278, 16755745, 16753955, 16752422, 16750888, 16749099, 13398052, 13396774, 16744243, 16742704, 16741166, 16739884, 16738345, 16736807, 16735269, 16733730, 13385753, 13384728, 16729371, 16727833, 16726295, 16725012, 16723474, 16721936, 16720397, 16718859, 13373959, 13372677, 16714500, 16712962, 16777215]  # Color table (Rainbow-striped)
          }
          frame "Jet" {
            w293 = u32[] [127, 131, 135, 139, 143, 147, 151, 155, 159, 163, 167, 171, 175, 179, 183, 187, 191, 195, 199, 203, 207, 211, 215, 219, 223, 227, 231, 235, 239, 243, 247, 251, 255, 1279, 2303, 3327, 4351, 5375, 6399, 7423, 8447, 9471, 10495, 11519, 12543, 13567, 14591, 15615, 16639, 17663, 18687, 19711, 20735, 21759, 22783, 23807, 24831, 25855, 26879, 27903, 28927, 29951, 30975, 31999, 33023, 34047, 35071, 36095, 37119, 38143, 39167, 40191, 41215, 42239, 43263, 44287, 45311, 46335, 47359, 48383, 49407, 50431, 51455, 52479, 53503, 54527, 55551, 56575, 57599, 58623, 59647, 60671, 61695, 62719, 63743, 64767, 131069, 393209, 655349, 917489, 1179629, 1441769, 1703909, 1966049, 2228189, 2490329, 2752469, 3014609, 3276749, 3538889, 3801029, 4063169, 4325309, 4587449, 4849589, 5111729, 5373869, 5636009, 5898149, 6160289, 6422429, 6684569, 6946709, 7208849, 7470989, 7733129, 7995269, 8257409, 8519549, 8781689, 9043829, 9305969, 9568109, 9830249, 10092389, 10354529, 10616669, 10878809, 11140949, 11403089, 11665229, 11927369, 12189509, 12451649, 12713789, 12975929, 13238069, 13500209, 13762349, 14024489, 14286629, 14548769, 14810909, 15073049, 15335189, 15597329, 15859469, 16121609, 16383749, 16645889, 16776192, 16775168, 16774144, 16773120, 16772096, 16771072, 16770048, 16769024, 16768000, 16766976, 16765952, 16764928, 16763904, 16762880, 16761856, 16760832, 16759808, 16758784, 16757760, 16756736, 16755712, 16754688, 16753664, 16752640, 16751616, 16750592, 16749568, 16748544, 16747520, 16746496, 16745472, 16744448, 16743424, 16742400, 16741376, 16740352, 16739328, 16738304, 16737280, 16736256, 16735232, 16734208, 16733184, 16732160, 16731136, 16730112, 16729088, 16728064, 16727040, 16726016, 16724992, 16723968, 16722944, 16721920, 16720896, 16719872, 16718848, 16717824, 16716800, 16715776, 16714752, 16713728, 16712704, 16711680, 16449536, 16187392, 15925248, 15663104, 15400960, 15138816, 14876672, 14614528, 14352384, 14090240, 13828096, 13565952, 13303808, 13041664, 12779520, 12517376, 12255232, 11993088, 11730944, 11468800, 11206656, 10944512, 10682368, 10420224, 10158080, 9895936, 9633792, 9371648, 9109504, 8847360, 8585216, 8323072]  # Jet(256)
          }
          frame "Rainbow_Wh" {
            w294 = u32[] [0, 262147, 589831, 851978, 1179662, 1441811, 1769495, 2031644, 2359328, 2621478, 2949163, 3276848, 3801147, 4194372, 4456520, 4522061, 4718673, 4849750, 5046363, 5177439, 5242980, 5374056, 5439597, 5505142, 5636218, 5767300, 5636232, 5701773, 5701777, 5701782, 5570714, 5505183, 5505187, 5505192, 5177521, 5111990, 5046458, 4980927, 4587720, 4456652, 4325585, 3932374, 3801306, 3604703, 3014888, 2818284, 2621681, 2359541, 2162938, 1638655, 1048831, 786687, 262399, 255, 1279, 4351, 5631, 6655, 7679, 9983, 11007, 12031, 13311, 16383, 17407, 18687, 21759, 23039, 24063, 25087, 27391, 28415, 29439, 30719, 32767, 34815, 36095, 39167, 40447, 41471, 42495, 44799, 45823, 46847, 48127, 50175, 51199, 55551, 56575, 57855, 58879, 59903, 62207, 63231, 64255, 65535, 65526, 65522, 65518, 65505, 65496, 65492, 65483, 65479, 65475, 65471, 65467, 65458, 65454, 65450, 65437, 65432, 65424, 65415, 65411, 65407, 65403, 65394, 65390, 65386, 65382, 65369, 65364, 65360, 65356, 65343, 65339, 65335, 65326, 65322, 65318, 65305, 65301, 65296, 65292, 65288, 65280, 589568, 851712, 1441536, 1703680, 1965824, 2817792, 3079936, 3407616, 3669760, 4194048, 4456192, 4783872, 5046016, 5897984, 6160128, 6422272, 7274240, 7536384, 7864064, 8126208, 8650496, 8912640, 9240320, 9502464, 10092288, 10616576, 10878720, 11730688, 11992832, 12320512, 12582656, 13106944, 13369088, 13696768, 13958912, 14548736, 14810880, 15924992, 16187136, 16449280, 16776960, 16775680, 16773632, 16772608, 16771328, 16770304, 16768256, 16766976, 16765952, 16762624, 16760576, 16759552, 16757248, 16756224, 16755200, 16753920, 16752896, 16750848, 16749568, 16748544, 16745216, 16744192, 16742144, 16739840, 16738816, 16737792, 16736512, 16734464, 16733440, 16732160, 16731136, 16727808, 16726784, 16725760, 16724736, 16721408, 16720384, 16719104, 16717056, 16716032, 16714752, 16711680, 16711680, 16711680, 16711680, 16711680, 16711680, 16711680, 16711680, 16711680, 16711680, 16711680, 16711680, 16711680, 16711680, 16711680, 16711680, 16711680, 16711680, 16777215, 16777215, 16777215, 16777215, 16777215, 16777215, 16777215, 16777215, 16777215, 16777215, 16777215, 16777215, 16777215, 16777215, 16777215, 16777215, 16777215, 16777215, 16777215, 16777215]  # Rainbow+White (237)
          }
          frame "Banded" {
            w295 = u32[] [6750846, 7013765, 7211659, 7409807, 7476371, 7411604, 7214997, 7017621, 6754453, 6490776, 6358685, 6226596, 6226092, 6226101, 6226109, 6227140, 6293961, 6296012, 6297806, 6233806, 5906635, 5512904, 4922053, 4199363, 3542212, 2950855, 2425550, 2031830, 1638622, 1376741, 1246954, 1314285, 1447407, 1975278, 2305771, 2372838, 2242272, 1783259, 1323992, 799448, 340956, 79842, 15849, 17905, 151543, 481786, 1009148, 1667324, 2193914, 2457333, 2523375, 2260968, 1801698, 1276895, 752607, 360418, 99816, 36335, 38390, 237307, 632574, 1158654, 1815550, 2275323, 2537717, 2471662, 2208487, 1683426, 1158879, 634847, 308451, 48362, 50673, 52728, 316924, 777214, 1302782, 1893373, 2352122, 2548212, 2481645, 2087398, 1628129, 1038303, 580576, 254949, 60394, 62189, 129520, 392688, 851694, 1441515, 2031078, 2423264, 2552791, 2419661, 2024898, 1499321, 974770, 516526, 190124, 60844, 62635, 129707, 458153, 982695, 1572516, 2161825, 2488475, 2552211, 2353800, 1893501, 1368177, 843623, 451166, 124759, 61010, 62797, 195401, 589383, 1113670, 1703494, 2227014, 2553410, 2551868, 2287665, 1827364, 1302294, 974603, 1040900, 1239041, 1699840, 2291200, 3013379, 3866121, 4783634, 5635611, 6355746, 6878502, 7073317, 7071521, 7004697, 6938385, 7069705, 7398403, 7858688, 8515840, 9172992, 9894916, 10550795, 11140627, 11599132, 11926051, 12055590, 11988261, 11855391, 11723032, 11788047, 11984904, 12510467, 13101824, 13759232, 14416129, 15006981, 15400460, 15728149, 15858974, 15857956, 15659558, 15395620, 15065886, 14736150, 14669582, 14800391, 15128322, 15587840, 16047616, 16441345, 16637958, 16703246, 16702743, 16570656, 16307237, 15846438, 15385379, 14924316, 14660116, 14658828, 14854661, 15182337, 15641344, 16100352, 16493826, 16690440, 16690192, 16690201, 16492833, 16163878, 15703078, 15242018, 14846235, 14647058, 14645003, 14840068, 15232513, 15690496, 16083200, 16410371, 16541193, 16541202, 16410139, 16213282, 15818789, 15292709, 14831136, 14434840, 14169616, 14166537, 14360579, 14686208, 15077888, 15404288, 15600132, 15665675, 15536665, 15342119, 15015986, 14558008, 14033211, 13507643, 13047097, 12848439, 12781367, 12911162, 13107263, 13303877, 13500748, 13501524, 13371996, 13177188, 12851050, 12393581, 11869549, 11278955, 10753384, 10293092, 9963875, 9765987, 9765220, 9764967, 9699434, 9634157, 9372526, 9111662, 8719469, 8261738]  # Banded(256)
          }
          frame "Seis" {
            w296 = u32[] [11206656, 11403264, 11599872, 11796480, 11993088, 12189696, 12386304, 12582912, 12779520, 12976128, 13172736, 13369344, 13565952, 13762560, 13959168, 14155776, 14352384, 14548992, 14745600, 14942208, 15138816, 15335424, 15532032, 15728640, 15925248, 16121856, 16318464, 16515072, 16711680, 16712448, 16713216, 16713984, 16714752, 16715520, 16716288, 16717056, 16717824, 16718592, 16719360, 16720128, 16720896, 16721664, 16722432, 16723200, 16723968, 16724736, 16725504, 16726272, 16727040, 16727808, 16728576, 16729344, 16730112, 16730880, 16731648, 16732416, 16733184, 16733952, 16734720, 16735488, 16736256, 16737024, 16737792, 16738560, 16739328, 16740096, 16740864, 16741632, 16742400, 16743168, 16743936, 16744448, 16745216, 16745984, 16746752, 16747520, 16748288, 16749056, 16749824, 16750592, 16751360, 16752128, 16752896, 16753664, 16754432, 16755200, 16755968, 16756736, 16757504, 16758272, 16759040, 16759808, 16760576, 16761344, 16762112, 16762880, 16763648, 16764416, 16765184, 16765952, 16766720, 16767488, 16768256, 16769024, 16769792, 16770560, 16771328, 16772096, 16772864, 16773632, 16774400, 16775168, 16775936, 16776704, 16776960, 16776960, 16776960, 16776960, 16776960, 16776960, 16776960, 16776960, 16776960, 16776960, 16776960, 16776960, 16776960, 16776960, 16776960, 16776960, 16776960, 16776960, 16776960, 16776960, 16776960, 16776960, 16776960, 16776960, 16776960, 16776960, 16776960, 16776960, 16645888, 16252673, 15924994, 15531779, 15138565, 14745350, 14352135, 14024456, 13631241, 13238026, 12844811, 12451596, 12123917, 11730702, 11337487, 10944272, 10551057, 10223378, 9830163, 9436948, 9043733, 8650518, 8322840, 7929625, 7536410, 7143195, 6749980, 6422301, 6029086, 5766944, 5570083, 5373222, 5176617, 4979756, 4717615, 4520753, 4324148, 4127287, 3930682, 3733821, 3471679, 3274818, 3078213, 2881352, 2684747, 2487886, 2225744, 2028883, 1832278, 1635417, 1438556, 1241950, 979553, 782948, 586087, 389482, 192620, 60784, 59509, 57979, 56704, 55173, 53642, 52367, 50836, 49305, 48030, 46499, 44968, 43694, 42163, 40888, 39357, 37826, 36551, 35020, 33489, 32214, 30684, 29409, 27878, 26347, 25072, 23541, 22010, 20735, 19965, 19195, 18426, 17912, 17142, 16372, 15603, 14833, 14319, 13549, 12780, 12010, 11240, 10726, 9957, 9187, 8417, 7647, 7134, 6364, 5594, 4824, 4055, 3541, 2771, 2001, 1232, 462]  # Seis(256)
          }
          frame "InvertSeis" {
            w297 = u32[] [462, 1232, 2001, 2771, 3541, 4055, 4824, 5594, 6364, 7134, 7647, 8417, 9187, 9957, 10726, 11240, 12010, 12780, 13549, 14319, 14833, 15603, 16372, 17142, 17912, 18426, 19195, 19965, 20735, 22010, 23541, 25072, 26347, 27878, 29409, 30684, 32214, 33489, 35020, 36551, 37826, 39357, 40888, 42163, 43694, 44968, 46499, 48030, 49305, 50836, 52367, 53642, 55173, 56704, 57979, 59509, 60784, 192620, 389482, 586087, 782948, 979553, 1241950, 1438556, 1635417, 1832278, 2028883, 2225744, 2487886, 2684747, 2881352, 3078213, 3274818, 3471679, 3733821, 3930682, 4127287, 4324148, 4520753, 4717615, 4979756, 5176617, 5373222, 5570083, 5766944, 6029086, 6422301, 6749980, 7143195, 7536410, 7929625, 8322840, 8650518, 9043733, 9436948, 9830163, 10223378, 10551057, 10944272, 11337487, 11730702, 12123917, 12451596, 12844811, 13238026, 13631241, 14024456, 14352135, 14745350, 15138565, 15531779, 15924994, 16252673, 16645888, 16776960, 16776960, 16776960, 16776960, 16776960, 16776960, 16776960, 16776960, 16776960, 16776960, 16776960, 16776960, 16776960, 16776960, 16776960, 16776960, 16776960, 16776960, 16776960, 16776960, 16776960, 16776960, 16776960, 16776960, 16776960, 16776960, 16776960, 16776960, 16776704, 16775936, 16775168, 16774400, 16773632, 16772864, 16772096, 16771328, 16770560, 16769792, 16769024, 16768256, 16767488, 16766720, 16765952, 16765184, 16764416, 16763648, 16762880, 16762112, 16761344, 16760576, 16759808, 16759040, 16758272, 16757504, 16756736, 16755968, 16755200, 16754432, 16753664, 16752896, 16752128, 16751360, 16750592, 16749824, 16749056, 16748288, 16747520, 16746752, 16745984, 16745216, 16744448, 16743936, 16743168, 16742400, 16741632, 16740864, 16740096, 16739328, 16738560, 16737792, 16737024, 16736256, 16735488, 16734720, 16733952, 16733184, 16732416, 16731648, 16730880, 16730112, 16729344, 16728576, 16727808, 16727040, 16726272, 16725504, 16724736, 16723968, 16723200, 16722432, 16721664, 16720896, 16720128, 16719360, 16718592, 16717824, 16717056, 16716288, 16715520, 16714752, 16713984, 16713216, 16712448, 16711680, 16515072, 16318464, 16121856, 15925248, 15728640, 15532032, 15335424, 15138816, 14942208, 14745600, 14548992, 14352384, 14155776, 13959168, 13762560, 13565952, 13369344, 13172736, 12976128, 12779520, 12582912, 12386304, 12189696, 11993088, 11796480, 11599872, 11403264, 11206656]  # InvertSeis(256)
          }
          frame "Jaisnd" {
            w298 = u32[] [3014783, 2949253, 2818187, 2621584, 2424982, 2228379, 2031776, 1769637, 1507497, 1245358, 917682, 655542, 327866, 190, 1218, 2757, 4041, 5580, 6863, 8402, 9941, 11480, 12763, 14301, 15840, 17378, 18916, 20198, 21736, 23274, 24556, 25837, 27375, 28656, 29938, 31219, 32500, 33781, 35062, 36343, 37368, 38649, 39673, 40698, 41723, 42747, 43772, 44796, 45821, 46589, 47613, 48381, 49406, 50174, 50942, 51710, 52478, 53502, 54270, 55038, 55806, 122110, 122878, 188926, 189695, 255999, 322303, 388607, 454911, 521215, 587519, 653823, 720127, 851966, 917499, 1048568, 1114101, 1245170, 1376239, 1441772, 1572841, 1703910, 1900515, 2031584, 2162653, 2293722, 2490327, 2621396, 2818001, 3014606, 3145676, 3342281, 3538886, 3735492, 3932097, 4194239, 4390845, 4587451, 4849593, 5046199, 5308341, 5570484, 5832626, 6029233, 6356912, 6619055, 6881199, 7143343, 7471022, 7733166, 8060847, 8388527, 8716208, 9043890, 9371571, 9764789, 10158007, 10485690, 10878908, 11337664, 11730884, 12189640, 12648397, 13172690, 13762520, 14352351, 15073256, 15990772, 16515059, 16318437, 16121818, 15990737, 15925192, 15859648, 15794105, 15794098, 15728556, 15728549, 15728543, 15794074, 15794068, 15859598, 15925129, 15925124, 15990655, 16056186, 16121717, 16252785, 16318316, 16383848, 16514916, 16580448, 16711515, 16776792, 16776276, 16775760, 16775244, 16774985, 16774469, 16773954, 16773439, 16772923, 16772408, 16771893, 16771378, 16770863, 16770093, 16769578, 16769063, 16768549, 16767778, 16767264, 16766750, 16765980, 16765465, 16764695, 16763925, 16763412, 16762642, 16761872, 16761103, 16760333, 16759564, 16758538, 16757769, 16757000, 16755975, 16755206, 16754181, 16753156, 16752131, 16751106, 16684546, 16683521, 16682497, 16681472, 16680192, 16679168, 16677888, 16676608, 16675328, 16674048, 16672768, 16671488, 16604672, 16603136, 16601856, 16600320, 16533248, 16531712, 16464640, 16463104, 16396032, 16328960, 16327168, 16260096, 16192768, 16125696, 16058368, 15991296, 15925252, 15859722, 15728657, 15663128, 15532062, 15466533, 15335467, 15204401, 15073335, 14942269, 14811203, 14680137, 14483535, 14352468, 14155865, 13959262, 13762659, 13566056, 13369452, 13172848, 12910708, 12714103, 12451962, 12189821, 11927679, 11665537, 11403394, 11075716, 10813572, 10485893, 10158212, 9830532, 9437315, 9109633, 8716415, 8323197]  # Jaisnd(256)
          }
          frame "TBD1" {
          }
        }
        n156 = property on="ImagePreview" class="IntGraph (strict)"("Color Table"=w288) -> ()  [unwired: 2 in, 2 out]
      }
      event "Start": Value Change {
        # "must check file exisance"
        n157 = event-data() -> ()  [unwired: 1 in, 1 out]
        n158 = while {
          tunnel: [w317] -> w304
          stop <- w318 stop-if-true
          n159 = Not A Number/Path/Refnum?(number/path/refnum="BioMAP file path") -> (NaN/Path/Refnum?=w315:bool)
          n160 = feedback #1(path "" ("selected path")) -> (w322:path)
          n161 = case shown="True" w315 {
            tunnel: w322 -> [_ w331]
            tunnel: [w324 w330] -> w320
            tunnel: [FALSE ("cancelled") w329] -> w319
            tunnel: "BioMAP file path" -> [w324 _]
            frame False {
            }
            frame True {
              n162 = Strip Path(path=w331) -> (stripped path=w326:path, name=w327:string)
              n163 = call "File Dialog2"("start path"=w326, "default name"=w327, "pattern (all files)"="*.img", "pattern label"="BioMAP Analyze v7.5") -> ("selected path"=w330:path, "cancelled"=w329:bool)  [unwired: 8 in, 2 out]
            }
          }
          n164 = case shown="True" w319 {
            tunnel: w320 -> [w334 _]
            tunnel: [w334 w342] -> w321
            tunnel: w322 -> [_ w342]
            tunnel: [w333 w341] -> w318
            tunnel: [w334 path "" ("selected path")] -> w317
            frame False {
              w332 = FALSE  # legacy
              n165 = Compound Arithmetic op=AND(invert w332, TRUE) -> (w333:bool)
              "Export File Path" <- w334
            }
            frame True {
              n166 = Two Button Dialog(message="No file saving?", 1:"No saving" ("F button name (\"Cancel\")"), 2:"Set filenare" ("T button name (\"OK\")")) -> (T button?=w336:bool)
              n167 = Not(x=w336) -> (.not. x?=w341:bool)
            }
          }
          n168 = feedback-in #1(w321) -> ()
        }
        n169 = property on="Start" class="Bool"("Visible"=FALSE) -> ()  [unwired: 2 in, 2 out]
        n170 = Bundle By Name(cluster=T15 {"State"=enum."SetPeakOI", "Para."=variant} ("element"), "Para."=w310) -> (w311:T15)
        n171 = Enqueue Element At Opposite End(queue=w313, element=w311) -> (queue out=w307:refnum<queue>)  [unwired: 2 in, 2 out]
        n172 = control-ref of="MaxiMass"() -> (w303:refnum<vi>)
        n173 = control-ref of="EnableBinning"() -> (w300:refnum<vi>)
        n174 = Bundle By Name(cluster=T15 {"State"=enum."Open", "Para."=variant} ("element"), "Para."=w304) -> (w305:T15)
        n175 = property class="DigNum (strict)"(reference=w303, "Visible"=FALSE) -> ()  [unwired: 1 in, 2 out]
        n176 = property class="Bool (strict)"(reference=w300, "Visible"=FALSE) -> ()  [unwired: 1 in, 2 out]
        n177 = Enqueue Element At Opposite End(queue=w307, element=w305) -> (queue out=w308:refnum<queue>)  [unwired: 2 in, 2 out]
      }
      event "m/z (Da)", "Integration Width (±Da)": Value Change {
        n178 = event-data() -> ()  [unwired: 1 in, 1 out]
        n179 = Enqueue Element(queue=w345, element=T15 {"State"=enum."Refresh_Profile", "Para."=variant}) -> (queue out=w344:refnum<queue>)  [unwired: 2 in, 2 out]
      }
    }
  }
  n180 = while {
    shift-right: [w365] -> _
    shift-left: w42 -> [w372]
    shift-right: [w364] -> _
    shift-left: _ -> [w371]
    tunnel: w35 -> [w370]
    tunnel: w48 -> [w368]
    tunnel: "Dynamic Params queue" -> [w361]
    shift-right: [w362] -> _
    shift-left: _ -> [w360]
    shift-right: [w359] -> _
    shift-left: _ -> [w358]
    tunnel: "Quit_UserEvent" -> [w357]
    shift-right: [w355] -> w22
    shift-left: w27 -> [w356]
    shift-right: [w351] -> _
    shift-left: w26 -> [w354]
    shift-right: [w352] -> _
    shift-left: T11 {"File Header"={"Start Position"=[], "StepWidth"=[], "Dimension"=[], "SpecLength"=0}, "mzCali."=[], "m/z_Array"=[], "SampleRate"=500000000.0, "TrigDelay"=0.0, "file refnum"=refnum, "file path"=path "", "PeakOI"=[], "Binning"={"Enable"=FALSE, "BinType"=enum."ByTime", "BinWidth"=0.0, "Maximum"=0.0, "Minimum"=0.0}} ("output cluster") -> [w353]
    border: w25 -> [_]
    border: ProcessStates."Initialize" -> [_]
    shift-right: [w348] -> _
    shift-left: _ -> [w347]
    i -> [w349]
    stop <- w363 stop-if-true
    n181 = Dequeue Element(queue=w370) -> (queue out=w366:refnum<queue>, element=w367:T15, error out=w369:errorcluster)  [unwired: 2 in, 1 out]
    n182 = Unbundle By Name(w367) -> ("State"=w350:T3)
    "State" <- w350
    n183 = case shown="No Error" w369 {
      tunnel: w372 -> [w396 w1348]
      tunnel: [w395 w1348] -> w365
      tunnel: w371 -> [w394 w1347]
      tunnel: [w393 w1347] -> w364
      tunnel: w368 -> [w392 _]
      tunnel: w350 -> [w391 _]
      tunnel: w367 -> [w390 _]
      tunnel: w366 -> [w389 _]
      tunnel: [w388 TRUE] -> w363
      tunnel: [w387 w1345] -> w362
      tunnel: w361 -> [w386 _]
      tunnel: w360 -> [w385 w1345]
      tunnel: [w384 w1344] -> w359
      tunnel: w358 -> [w383 w1344]
      tunnel: w357 -> [w382 _]
      tunnel: w356 -> [w381 w1343]
      tunnel: [w375 w1343] -> w355
      tunnel: w354 -> [w380 w1341]
      tunnel: w353 -> [w379 w1342]
      tunnel: [w378 w1342] -> w352
      tunnel: [w377 w1341] -> w351
      tunnel: [w374 w1340] -> w348
      tunnel: w347 -> [w373 w1340]
      frame No Error {
        n184 = case "Proc. Core" shown="\"Flush\"" w391 {
          selector: w391 -> [_ w495 w523 _ w769 w817 _ _ _ _ _ _ _ _ _ _]
          tunnel: w396 -> [w413 w432 w537 w582 w750 w822 w830 w1004 w1026 w1057 w1059 w1088 w1133 w1143 w1328 w1339]
          tunnel: [w399 w502 w519 w583 w750 w822 w830 w1004 w1026 w1057 w1059 w1088 w1133 w1143 w1328 w1339] -> w395
          tunnel: [w419 0 w517 w617 w760 w814 w847 w1008 w1025 w1056 w1074 w1102 w1132 w1189 w1319 w1338] -> w393
          tunnel: w394 -> [w419 _ w517 w617 w729 w814 w847 w1008 w1025 w1056 w1074 w1102 w1132 w1189 w1319 w1338]
          tunnel: w392 -> [_ _ _ w613 w739 _ _ _ w1023 _ _ _ _ _ _ _]
          tunnel: w390 -> [_ w458 w525 w615 w770 w818 _ _ _ w1048 _ _ _ w1182 w1327 _]
          tunnel: w389 -> [_ w496 w526 w616 w771 w819 w832 _ _ _ _ _ _ _ _ _]
          tunnel: [_ _ _ _ _ _ _ _ TRUE _ _ _ _ _ _ _] -> w388
          tunnel: [w418 w481 w521 w614 w733 w816 w844 w1002 w1022 w1051 w1073 w1101 w1131 w1185 w1320 w1337] -> w387
          tunnel: w386 -> [_ _ w528 _ _ _ _ _ w1015 _ _ _ _ _ _ _]
          tunnel: w385 -> [w418 _ w521 w614 w734 w816 w844 w1002 w1022 w1051 w1073 w1101 w1131 w1185 w1320 w1337]
          tunnel: [w417 w491 w518 w597 w768 w815 w843 w994 w1021 w1055 w1072 w1100 w1130 w1188 w1318 w1336] -> w384
          tunnel: w383 -> [w417 _ w518 w597 w768 w815 w843 w994 w1021 w1055 w1072 w1100 w1130 w1188 w1318 w1336]
          tunnel: w382 -> [_ _ _ _ _ _ _ _ w1020 _ _ _ _ _ _ _]
          tunnel: w381 -> [w416 _ w516 w612 _ w813 w842 w988 w1010 w1054 w1071 w1099 w1129 w1187 w1329 w1335]
          tunnel: [w416 w469 w515 w612 w766 w813 w842 w988 w1011 w1054 w1071 w1099 w1129 w1187 w1329 w1335] -> w376
          tunnel: w380 -> [w402 w433 w513 w609 w767 w811 w841 w989 w1013 w1052 w1069 w1097 w1128 w1186 w1331 w1333]
          tunnel: w379 -> [w415 w467 w514 w584 w728 w812 w829 w990 w1014 w1053 w1070 w1098 w1117 w1142 w1325 w1334]
          tunnel: [w414 w470 w514 w584 w728 w812 w829 w990 w1014 w1053 w1070 w1098 w1117 w1142 w1330 w1334] -> w378
          tunnel: [w402 w433 w513 w610 w767 w811 w841 w989 w1013 w1052 w1069 w1097 w1128 w1186 w1331 w1333] -> w377
          tunnel: [w397 w434 w512 w581 w726 w810 w823 w986 w1009 w1030 w1061 w1089 w1116 w1140 w1317 w1332] -> w374
          tunnel: w373 -> [w397 _ w512 w581 w727 w810 w823 w986 w1009 w1030 w1061 w1089 w1116 w1140 w1317 w1332]
          frame "Initialize" {
            w398 = 0  # Scan#, should not be reset to 0 in "open", for 3D imaging.
            n185 = Unbundle By Name(w413) -> ("File Header.SpecLength"=w409:i32, "File Header"=w407:T12, "mzCali."=w412:dbl[], "SampleRate"=w410:T13, "TrigDelay"=w411:dbl)
            n186 = disable-structure shown="Disabled" {
              frame Disabled {
                w420 = u32[] [0, 0, 12517567, 12320960, 12189888, 12058817, 11927746, 11731139, 11600067, 9175197, 9044125, 11141318, 11010246, 10813639, 10682568, 10551497, 10354890, 10223818, 10092747, 7930019, 7798948, 9633997, 9502926, 9306319, 9175248, 9044176, 8847569, 8716498, 8585427, 6750377, 6619306, 8126677, 7995606, 7798999, 7667927, 7536856, 7340249, 7209178, 7078106, 5505199, 5374128, 6619357, 6488285, 6291678, 6160607, 6029536, 5832929, 5701857, 5570786, 4325557, 4194486, 5112036, 4980965, 4784358, 4653287, 4522215, 4325608, 4194537, 4063466, 3080380, 3014844, 3604716, 3408109, 3277038, 3277038, 3145966, 3014895, 2818288, 2687217, 2556145, 1900738, 1769666, 2097396, 1900789, 1769717, 1638646, 1507575, 1310968, 1179896, 1048825, 721096, 590024, 590075, 393468, 262397, 131326, 255, 1791, 3327, 4863, 5068, 6348, 9471, 11007, 12543, 14079, 15615, 17151, 18687, 20223, 17612, 18636, 25087, 26623, 28159, 29695, 31231, 32767, 34303, 35839, 29900, 31180, 40447, 41983, 43775, 45311, 46847, 48383, 49919, 51455, 42444, 43724, 56063, 57599, 59135, 60671, 62207, 63743, 65535, 65528, 52418, 52413, 65510, 65504, 65498, 65492, 65486, 65480, 65474, 65468, 52369, 52364, 65449, 65443, 65437, 65431, 65425, 65419, 65413, 65407, 52321, 52316, 65389, 65383, 65377, 65371, 65364, 65358, 65352, 65346, 52272, 52267, 65328, 65322, 65316, 65310, 65304, 65298, 65292, 65286, 52224, 314368, 851712, 1244928, 1638144, 2031360, 2424576, 2817792, 3211008, 3604224, 3197952, 3525632, 4783872, 5177088, 5635840, 6029056, 6422272, 6815488, 7208704, 7601920, 6409216, 6736896, 6736896, 8781568, 9174784, 9568000, 9961216, 10354432, 10747648, 11206400, 11599616, 9554944, 9882624, 12779264, 13172480, 13565696, 13958912, 14352128, 14745344, 15138560, 15531776, 12766208, 13093888, 16776960, 16775170, 16773637, 16771847, 16770314, 16768780, 16766991, 16765457, 13411088, 13409810, 16760601, 16758812, 16757278, 16755745, 16753955, 16752422, 16750888, 16749099, 13398052, 13396774, 16744243, 16742704, 16741166, 16739884, 16738345, 16736807, 16735269, 16733730, 13385753, 13384728, 16729371, 16727833, 16726295, 16725012, 16723474, 16721936, 16720397, 16718859, 13373959, 13372677, 16714500, 16712962, 16777215]  # Color table (Rainbow-striped)
                # "Probably to be deleted"
                n187 = property on="ImagePreview" class="IntGraph (strict)"("Color Table"=w420) -> ()  [unwired: 2 in, 2 out]
              }
              frame Enabled {
              }
            }
            n188 = in-place "Compensate error in float-point number calculation" {
              n189 = in-place-cluster #2(w407) -> ("StepWidth"=w421:dbl[], "Start Position"=w426:dbl[])
              n190 = Index Array(array=w421) -> (element=w425:dbl)  [unwired: 1 in]
              n191 = Multiply(x=w425, y=0.001) -> (x*y=w423:dbl)
              n192 = in-place {
                in-place-border: w423 -> [w428]
                n193 = in-place-array #3(w426, 0) -> (w429:dbl)
                n194 = Subtract(x=w429, y=w428) -> (x-y=w430:dbl)
                n195 = in-place-array #3(w430) -> (w427:dbl[])  [unwired: 1 out]
              }
              n196 = in-place-cluster #2("StepWidth"=w421, "Start Position"=w427) -> (w406:T12)
            }
            n197 = Subtract "Gage DAQ does not always gives same length spectrum"(x=w409, y=64) -> (x-y=w400:i32)
            n198 = call "CalcMzArray.vi"("TrigDelay"=w411, "Sample Rate"=w410, "Depth"=w400, "mzCali. (a/b/c)"=w412) -> ("mzArray"=w401:dbl[])  [unwired: 7 in]
            n199 = Bundle By Name(cluster=w413, "Scan#"=w398) -> (w399:T16)
            n200 = Bundle By Name(cluster=w415, "Binning.BinType"=BinType."ByMass", "Binning.BinWidth"=0.1, "Binning.Minimum"=0.0, "File Header.SpecLength"=w400, "m/z_Array"=w401, "File Header"=w406, "mzCali."=w412, "SampleRate"=w410, "TrigDelay"=w411) -> (w414:T11)
          }
          frame "Open" {
            (unwired) T22 {"queue out"=refnum, "queue out"=refnum} ("output cluster")
            w476 = "ActionCallBack" ("name (unnamed)")
            # "Save Header + MzArray first.\nIn case of program crash, \nBioMAP v3.8+ will load partial file just fine."
            # "8192x32KB*4 = 1GB\n!! attention:\nshould be big"
            n201 = Increment(x=w495) -> (x+1=w497:T3)
            n202 = Unbundle By Name(w432) -> ("File Header.SpecLength"=w444:i32, "File Header.Dimension"=w438:i32[], "mzCali."=w440:dbl[], "SampleRate"=w441:T13, "TrigDelay"=w442:dbl)
            n203 = Bundle By Name(cluster=w458, "State"=w497) -> (w498:T15)
            n204 = Unbundle By Name(w458) -> ("Para."=w457:variant)
            n205 = Enqueue Element(queue=w496, element=w498) -> ()  [unwired: 2 in, 3 out]
            n206 = Variant To Data(type=path "" ("selected path"), Variant=w457) -> (data=w449:path, error out=w453:errorcluster)  [unwired: 1 in]
            n207 = call "CalcMzArray.vi"("TrigDelay"=w442, "Sample Rate"=w441, "Depth"=w444, "mzCali. (a/b/c)"=w440) -> ("mzArray"=w443:dbl[])  [unwired: 7 in]
            n208 = Initialize Array(sgl 0.0 ("element"), w444) -> (w436:sgl[])
            n209 = Bundle By Name(cluster=w432, "mzArray"=w443) -> (w431:T16)
            n210 = Open/Create/Replace File(file path (use dialog)=w449, error in=w453, operation (0:open)=T21."create", access (0:read/write)=enum16{"read/write", "read-only", "write-only"}."write-only") -> (refnum out=w447:refnum<file>, error out=w451:errorcluster)  [unwired: 2 in, 1 out]
            n211 = Obtain Queue(max queue size (-1, unlimited)=4096, name (unnamed)="BeamProfiling_Buffer", element data type=T24 {"SampleRate"=0.0, "TrigDelay"=0.0, "SpecLength"=0.0, "DAQ_Range"=0.0, "Average#"=0, "Position"=[], "Spectrum"=[], "Calibr."=[], "Pressure"=0.0, "Desp_LaserEnergy"=0.0, "PI_LaserEnergy"=0.0, "Voltages Table"=[], "ProcMode"=enum."None", "Threshold"=0.0, "Comment"="", "TickCount"=0.0, "Time Stamp"=timestamp(0 s since 1904-01-01)} ("Signal Segment")) -> (queue out=w491:refnum<queue>, error out=w490:errorcluster)  [unwired: 2 in, 1 out]
            n212 = Obtain Queue(name (unnamed)=w476, element data type=w476) -> (queue out=w473:refnum<queue>)  [unwired: 3 in, 2 out]
            n213 = Index Array(array=w438, index=2) -> ()  [unwired: 1 out]
            n214 = Bundle By Name(cluster=w433, "Spectra"=w436) -> (w435:T10)
            n215 = case shown="Error" w451 {
              selector: w451 -> [_ w510]
              tunnel: [_ w510] -> w450
              tunnel: w449 -> [w504 w506]
              tunnel: [w504 w506] -> w448
              tunnel: w447 -> [w503 w505]
              tunnel: [w503 w505] -> w446
              frame No Error {
              }
              frame Error {
                n216 = Two Button Dialog(message="Error when create image file.", 1:"No saving" ("F button name (\"Cancel\")"), 2:"Ignore" ("T button name (\"OK\")")) -> ()  [unwired: 1 out]
              }
            }
            n217 = Unbundle By Name(w431) -> ("ControlRefs.ProcCore_CtrlQueue"=w492:refnum<queue>)
            n218 = Bundle(cluster=T22 {"queue out"=refnum, "queue out"=refnum}, "queue out"=w491, "queue out"=w473) -> (w482:T22)
            n219 = Initialize Array(w435) -> (w434:T29)  [unwired: 1 in]
            n220 = Bundle By Name(cluster=T23 {"Command"=enum."SetWriterRef", "Params"=variant} ("element"), "Command"=ProcessStates."SetWriterRef", "Params"=w482) -> (w500:T23)
            n221 = Enqueue Element "Set Data queue"(queue=w492, element=w500, error in (no error)=w490) -> (queue out=w485:refnum<queue>, error out=w475:errorcluster)  [unwired: 1 in, 1 out]
            n222 = Dequeue Element(queue=w473, error in (no error)=w475) -> (error out=w474:errorcluster)  [unwired: 1 in, 3 out]
            n223 = Bundle By Name(cluster=T23 {"Command"=enum."SetWriterRef", "Params"=variant} ("element"), "Command"=ProcessStates."StartSave") -> (w487:T23)
            n224 = Unbundle By Name(w467) -> ("Binning.BinWidth"=w463:dbl, "Binning.Minimum"=w464:dbl, "m/z_Array"=w465:dbl[], "Binning.BinType"=w466:T1)
            n225 = Enqueue Element "Start Send Data"(queue=w485, element=w487, error in (no error)=w474) -> (error out=w484:errorcluster)  [unwired: 1 in, 2 out]
            n226 = Unbundle By Name(w467) -> ("File Header.Dimension"=w479:i32[])
            n227 = call <vilib>:"Clear Errors.vi"("error in (no error)"=w484) -> ()  [unwired: 6 in, 1 out]
            n228 = Bundle By Name(cluster=w467, "Binning.Maximum"="MaxiMass", "Binning.Enable"="EnableBinning", "file path"=w448, "file refnum"=w446) -> (w470:T11)
            n229 = Index Array(array=w479) -> (element #1=w478:i32, element #2=w477:i32)  [unwired: 2 in]
            n230 = call "SpectrumBinning_NoGraph.vi"("XScale.Maximum"="MaxiMass", "BinType"=w466, "BinWidth"=w463, "Enable"="EnableBinning", "Signal"=w465, "m/z Array"=w465, "XScale.Minimum"=w464) -> ("m/z Array"=w462:dbl[])  [unwired: 2 in, 2 out]
            n231 = Initialize Array "<= Potential Insufficient Memory Source"(sgl -1.0, w478, w477, 32 ("dimension size")) -> (w481:sgl[][][])
            n232 = Unbundle By Name(w450) -> ("status"=w452:bool)
            n233 = Array Size(array=w462) -> (size(s)=w461:i32)
            n234 = Bundle By Name(cluster=w470, "File Header.SpecLength"=w461, "m/z_Array"=w462) -> (w468:T11)
            n235 = Not(x=w452) -> (.not. x?=w445:bool)
            n236 = call "WriteHeader+MzArray(AnalyzeV75).vi"("error in (no error)"=w450, "ImageConvParams"=w468) -> ("error out"=w469:errorcluster)  [unwired: 9 in]
            n237 = Bundle By Name(cluster=w431, "Save?"=w445) -> (w502:T16)
          }
          frame "PrepScanParams" {
            n238 = Increment(x=w523) -> (x+1=w522:T3)
            n239 = Bundle By Name(cluster=w525, "State"=w522) -> (w524:T15)
            n240 = Unbundle By Name(w537) -> ("Scan#"=w529:i32)
            n241 = Enqueue Element(queue=w526, element=w524) -> ()  [unwired: 2 in, 3 out]
            n242 = Equal To 0?(x=w529) -> (x = 0?=w538:bool)
            n243 = case shown="False" w538 {
              tunnel: w537 -> [w551 w578]
              tunnel: [w541 w574] -> w534
              tunnel: [w545 w577] -> w533
              tunnel: [w544 w576] -> w532
              tunnel: [w543 w575] -> w531
              tunnel: w529 -> [_ w559]
              tunnel: w517 -> [_ _]
              tunnel: [0 w555] -> w511
              frame True {
                w540 = 0
                # "Initial scan, stick to orignal parameter"
                n244 = Unbundle By Name(w551) -> ("HighSpeed"=w544:dbl, "ScanSpeed"=w543:dbl, "File Header"=w546:T12)
                n245 = Unbundle By Name(w546) -> ("Start Position"=w541:dbl[], "StepWidth"=w549:dbl[], "Dimension"=w550:i32[])
                n246 = Index Array(array=w549, index=w540) -> (element=w548:dbl)
                n247 = Index Array(array=w550, index=w540) -> (element=w547:i32)
                n248 = Multiply(x=w548, y=w547) -> (x*y=w542:dbl)
                n249 = in-place {
                  in-place-border: w542 -> [w553]
                  n250 = in-place-array #4(w541, w540) -> (w554:dbl)
                  n251 = Add(x=w554, y=w553) -> (x+y=w552:dbl)
                  n252 = in-place-array #4(w552) -> (w545:dbl[])  [unwired: 1 out]
                }
              }
              frame False {
                w556 = 1
                w565 = 0 ("index")
                n253 = Unbundle By Name(w578) -> ("HighSpeed"=w576:dbl, "ScanSpeed"=w575:dbl, "File Header"=w567:T12)
                n254 = Unbundle By Name(w567) -> ("Start Position"=w560:dbl[], "StepWidth"=w572:dbl[], "Dimension"=w573:i32[])
                n255 = Index Array(array=w560, index #1=w565, index #2=w556) -> (element #1=w571:dbl, element #2=w562:dbl)
                n256 = Index Array(array=w572, index #1=w565, index #2=w556) -> (element #1=w569:dbl, element #2=w564:dbl)
                n257 = Index Array(array=w573, index #1=w565, index #2=w556) -> (element #1=w568:i32, element #2=w558:i32)
                n258 = Quotient & Remainder "Circle Y #"(x=w559, y=w558) -> (x-y*floor(x/y)=w557:i32, floor(x/y)=w555:i32)
                n259 = Multiply(x=w569, y=w568) -> (x*y=w570:dbl)
                n260 = Multiply(x=w564, y=w557) -> (x*y=w563:dbl)
                n261 = Add "X"(x=w571, y=w570) -> (x+y=w566:dbl)
                n262 = Add "Y"(x=w562, y=w563) -> (x+y=w561:dbl)
                n263 = in-place {
                  in-place-border: w566 -> [w580]
                  in-place-border: w561 -> [w579]
                  # "X"
                  # "Y"
                  n264 = in-place-array #5(w560, w556) -> ()  [unwired: 1 out]
                  n265 = in-place-array #6(w560, w565, w556) -> ()  [unwired: 2 out]
                  n266 = in-place-array #5(w579) -> (w574:dbl[])  [unwired: 1 out]
                  n267 = in-place-array #6(w580, w579) -> (w577:dbl[])  [unwired: 2 out]
                }
              }
            }
            n268 = Bundle By Name(cluster=T26 {"Line Start"=[], "Line End"=[], "HighSpeed"=0.0, "ScanSpeed"=0.0, "KeepStill(ms)"=0, "InstruParams"=[]}, "HighSpeed"=w532, "ScanSpeed"=w531, "Line Start"=w534, "Line End"=w533, "KeepStill(ms)"=u32 0 ("Wait(ms)")) -> (w527:T26)
            n269 = Increment(x=w529) -> (x+1=w536:i32)
            n270 = Enqueue Element "Send scan params"(queue=w528, element=w527) -> (error out=w520:errorcluster)  [unwired: 2 in, 2 out]
            n271 = Bundle By Name(cluster=w537, "Scan#"=w536, "Z_Counter"=w511) -> (w519:T16)
            n272 = Merge Errors(w520, w516) -> (w515:errorcluster)
            n273 = call <vilib>:"Clear Errors.vi"("error in (no error)"=w520) -> ()  [unwired: 6 in, 1 out]
          }
          frame "WaitData" {
            w604 = u32 73  # A prime number to avoid artifact
            # "Only for file conversion\nNothing to do with online conversion"
            # "Potential dead lock"
            # "Need EOF detection, \nAnd set Y Dimension to current value"
            n274 = Dequeue Element "WaitSpectra"(queue=w597) -> (element=w618:T24)  [unwired: 2 in, 3 out]
            n275 = Unbundle By Name(w618) -> ("TickCount"=w591:dbl, "Position"=w602:dbl[], "Spectrum"=w595:sgl[], "Average#"=w593:i32, "Comment"=w588:string)
            n276 = Search and Replace String(input string=w588, search string="EOF" ("y")) -> (number of replacements=w586:i32)  [unwired: 6 in, 3 out]
            n277 = String Subset(string=w588, length (rest)=2 ("length (rest)")) -> (substring=w592:string)  [unwired: 1 in]
            n278 = Type Cast(type=ProcessStates."StartOfLine", x=w592) -> (*(type *) &x=w599:T9)
            n279 = Unbundle By Name(w584) -> ("File Header.Start Position"=w600:dbl[], "File Header.StepWidth"=w601:dbl[])
            n280 = Greater Than 0?(x=w586) -> (x > 0?=w585:bool)
            n281 = Select(t=ProcessStates."Quit", s=w585, f=w599) -> (s? t:f=w590:T9)
            n282 = feedback-in #7(w590) -> ()
            n283 = feedback #7() -> (w598:T9)
            n284 = Multiply(x=w595, y=w593) -> (x*y=w594:sgl[])
            n285 = case "Average Spectra in a single pixel" shown="Default" w590 {
              tunnel: w616 -> [w638 w655 w667 w697]
              tunnel: w613 -> [w625 w652 w665 w695]
              tunnel: w615 -> [_ _ w666 w696]
              tunnel: w609 -> [w635 w651 _ w668]
              tunnel: [_ _ _ w694] -> w610
              tunnel: [w634 w650 _ w693] -> w603
              tunnel: w594 -> [_ _ _ w680]
              tunnel: w602 -> [_ _ _ w679]
              tunnel: w601 -> [_ _ _ w678]
              tunnel: w600 -> [_ _ _ w677]
              tunnel: w598 -> [_ _ _ w675]
              tunnel: [_ _ _ w673] -> _
              tunnel: w593 -> [_ _ _ w670]
              tunnel: w591 -> [_ _ _ _]
              tunnel: [w626 w644 w661 w669] -> w583
              tunnel: w582 -> [w626 w643 w661 w669]
              frame "EndOfLine" {
                # "for debug"
                # "End of Line"
                n286 = Unbundle By Name(w635) -> ("Average"=w636:i32, "Spectra"=w637:sgl[])
                n287 = Enqueue Element At Opposite End(queue=w638, element=T15 {"State"=enum."Flush", "Para."=variant}) -> ()  [unwired: 2 in, 3 out]
                n288 = To Single Precision Float(number=w637) -> (single precision float=w633:sgl[])
                n289 = To Single Precision Float(number=w636) -> (single precision float=w632:sgl)
                n290 = Divide(x=w633, y=w632) -> (x/y=w634:sgl[])
                n291 = Bundle By Name(cluster=w635, "Average"=w636, "Spectra"=w634) -> (w631:T10)
                n292 = Enqueue Element(queue=w625, element=w631) -> ()  [unwired: 2 in, 3 out]
                n293 = feedback #8(0) -> (w628:i32)
                n294 = Increment(x=w628) -> (x+1=w627:i32)
                "#EOL" <- w627
                n295 = feedback-in #8(w627) -> ()
              }
              frame "Quit" {
                # "Does NOT handle 3D image !!"
                # "For incomplete files"
                # "End of File detected (Only for incomplete file)"
                n296 = Unbundle By Name(w651) -> ("Average"=w653:i32, "Spectra"=w654:sgl[])
                n297 = disable-structure shown="Enabled" {
                  disable-tunnel: w655 -> [w659 w660]
                  disable-tunnel: [w658 w660] -> w645
                  frame Disabled {
                    n298 = Enqueue Element At Opposite End(queue=w659, element=T15 {"State"=enum."Close", "Para."=variant}) -> (queue out=w658:refnum<queue>)  [unwired: 2 in, 2 out]
                  }
                  frame Enabled {
                  }
                }
                n299 = To Single Precision Float(number=w654) -> (single precision float=w649:sgl[])
                n300 = To Single Precision Float(number=w653) -> (single precision float=w648:sgl)
                n301 = Unbundle By Name(w643) -> ("File Header.Dimension"=w642:i32[], "Scan#"=w639:i32)
                n302 = Divide(x=w649, y=w648) -> (x/y=w650:sgl[])
                n303 = Bundle By Name(cluster=w651, "Average"=w653, "Spectra"=w650) -> (w647:T10)
                n304 = Enqueue Element(queue=w652, element=w647) -> ()  [unwired: 2 in, 3 out]
                n305 = in-place {
                  in-place-border: w639 -> [w656]
                  n306 = in-place-array #9(w642, 1) -> ()  [unwired: 1 out]
                  n307 = in-place-array #9(w656) -> (w641:i32[])  [unwired: 1 out]
                }
                n308 = Enqueue Element At Opposite End(queue=w645, element=T15 {"State"=enum."Flush", "Para."=variant}) -> ()  [unwired: 2 in, 3 out]
                n309 = Bundle By Name(cluster=w643, "File Header.Dimension"=w641) -> (w644:T16)
              }
              frame "StartOfLine" {
                # "New Line"
                n310 = Enqueue Element "Implied \"WaitData\""(queue=w667, element=w666) -> ()  [unwired: 2 in, 3 out]
                n311 = Flush Queue(queue=w665) -> ()  [unwired: 1 in, 3 out]
                n312 = feedback #10(0) -> (w663:i32)
                n313 = Increment(x=w663) -> (x+1=w662:i32)
                "#SOL" <- w662
                n314 = feedback-in #10(w662) -> ()
              }
              frame Default {
                # "cluster initialize?"
                # "Legacy"
                # "Normal Spectra"
                n315 = Index Array(array=w677) -> (element #1=w688:dbl, element #2=w689:dbl)  [unwired: 2 in]
                n316 = Index Array(array=w678) -> (element #1=w690:dbl, element #2=w691:dbl)  [unwired: 2 in]
                n317 = Index Array(array=w679) -> (element #1=w674:dbl, element #2=w692:dbl)  [unwired: 2 in]
                n318 = Enqueue Element "\"WaitData\" \nImplied"(queue=w697, element=w696) -> ()  [unwired: 2 in, 3 out]
                n319 = Subtract "Y"(x=w692, y=w689) -> (x-y=w685:dbl)
                n320 = Subtract "X"(x=w674, y=w688) -> (x-y=w686:dbl)
                n321 = Divide(x=w685, y=w691) -> (x/y=w684:dbl)
                n322 = Divide(x=w686, y=w690) -> (x/y=w687:dbl)
                n323 = Round Toward -Infinity(1:w687) -> (0:w682:dbl)
                n324 = Round Toward -Infinity(1:w684) -> (0:w683:dbl)
                n325 = To Long Integer(number=w682) -> (32bit integer=w671:i32)
                n326 = To Long Integer(number=w683) -> (32bit integer=w672:i32)
                n327 = call-poly <userlib>:"Data Changed__ogtk.vi"("I32"=w672) -> ("Changed"=w673:bool)
                n328 = Bundle By Name(cluster=w668, "X (Img)"=w671, "Y (Img)"=w672, "Spectra"=w680, "Average"=w670) -> (w681:T10)
                n329 = call-poly <userlib>:"Data Changed__ogtk.vi"("I32"=w671) -> ("Changed"=w676:bool)
                n330 = case shown="False" w676 {
                  tunnel: w695 -> [_ w718]
                  tunnel: w668 -> [w702 w714]
                  tunnel: [w703 w716] -> w694
                  tunnel: w681 -> [w701 w716]
                  tunnel: [w700 w713] -> w693
                  tunnel: w675 -> [_ w711]
                  frame False {
                    # "To be averaged"
                    n331 = Unbundle By Name(w701) -> ("Spectra"=w698:sgl[], "Average"=w699:i32)
                    n332 = in-place {
                      in-place-border: w698 -> [w709]
                      in-place-border: w699 -> [w707]
                      in-place-border: [w706] -> w700
                      n333 = in-place-cluster #11(w702) -> ("Spectra"=w705:sgl[], "Average"=w704:i32)
                      n334 = Compound Arithmetic op=ADD(w705, w709) -> (w706:sgl[])
                      n335 = Compound Arithmetic op=ADD(w704, w707) -> (w708:i32)
                      n336 = in-place-cluster #11("Spectra"=w706, "Average"=w708) -> (w703:T10)
                    }
                  }
                  frame True {
                    # "First one of a pixel"
                    n337 = Unbundle By Name(w714) -> ("Average"=w715:i32, "Spectra"=w719:sgl[])
                    "# average" <- w715
                    n338 = Not Equal?(x=ProcessStates."StartOfLine", y=w711) -> (x != y?=w710:bool)
                    n339 = To Single Precision Float(number=w719) -> (single precision float=w721:sgl[])
                    n340 = To Single Precision Float(number=w715) -> (single precision float=w720:sgl)
                    n341 = Divide(x=w721, y=w720) -> (x/y=w713:sgl[])
                    n342 = Bundle By Name(cluster=w714, "Average"=w715, "Spectra"=w713) -> (w717:T10)
                    n343 = case shown="True" w710 {
                      tunnel: w718 -> [_ w723]
                      tunnel: w717 -> [_ w722]
                      frame False {
                      }
                      frame True {
                        n344 = Enqueue Element ("Push previous to stack")(queue=w723, element=w722) -> ()  [unwired: 2 in, 3 out]
                      }
                    }
                  }
                }
              }
            }
            n345 = Tick Count (ms)() -> (millisecond timer value=w605:u32)
            n346 = Less?(x=w604, y=w605) -> (x < y?=w606:bool)
            n347 = feedback #12() -> (w607:u32)
            n348 = case "raw MS refresh" shown="True" w606 {
              tunnel: w603 -> [_ w623]
              tunnel: w605 -> [_ w624]
              tunnel: [w619 w624] -> w608
              tunnel: w607 -> [w619 _]
              tunnel: w584 -> [_ w621]
              frame False {
              }
              frame True {
                n349 = Unbundle By Name(w621) -> ("m/z_Array"=w622:dbl[])
                n350 = Bundle("m/z_Array"=w622, w623) -> (→"MS (Raw)":cluster{"m/z_Array":dbl[], sgl[]})  [unwired: 1 in]
              }
            }
            n351 = feedback-in #12(w608) -> ()
          }
          frame "Flush" {
            # "Need to be re-written"
            n352 = Preview Queue Element(queue=w771, timeout in ms (-1)=0) -> (queue out=w759:refnum<queue>, element=w756:T15, timed out?=w751:bool, error out=w758:errorcluster)  [unwired: 1 in]
            n353 = Not Equal?(x=T15 {"State"=enum."Close", "Para."=variant}, y=w756) -> (x != y?=w755:cluster{"State":bool, "Para.":bool})
            n354 = Unbundle By Name(w755) -> ("State"=w754:bool)
            n355 = Or(x=w754, y=w751) -> (x .or. y?=w752:bool)
            n356 = case shown="False" w752 {
              tunnel: w770 -> [_ w807]
              tunnel: w769 -> [_ w806]
              tunnel: [w801 w805] -> w765
              tunnel: [w800 w804] -> w764
              tunnel: w759 -> [w801 w803]
              tunnel: w758 -> [w800 w802]
              frame False {
              }
              frame True {
                n357 = Increment(x=w806) -> (x+1=w808:T3)
                n358 = Bundle By Name(cluster=w807, "State"=w808) -> (w809:T15)
                n359 = Enqueue Element(queue=w803, element=w809, error in (no error)=w802) -> (queue out=w805:refnum<queue>, error out=w804:errorcluster)  [unwired: 1 in, 1 out]
              }
            }
            n360 = property on="PeakOI #" class="DigNum (strict)"() -> ("Value"=w761:i32)  [unwired: 2 in, 2 out]
            n361 = Unbundle By Name(w728) -> ("Binning.Maximum"=w743:dbl, "Binning.BinWidth"=w742:dbl, "Binning.Enable"=w737:bool, "Binning.Minimum"=w741:dbl, "m/z_Array"=w738:dbl[], "Binning.BinType"=w740:T1)
            n362 = Unbundle By Name(w750) -> ("Z_Counter"=w732:i32, "InfoBarRef."=w749:refnum<vi>)
            n363 = Bundle By Name(cluster=T15 {"State"=enum."Refresh_Image", "Para."=variant} ("element"), "Para."=w761) -> (w762:T15)
            n364 = Enqueue Element(queue=w765, element=w762, error in (no error)=w764) -> (error out=w736:errorcluster)  [unwired: 1 in, 2 out]
            n365 = Get Queue Status(queue=w739, error in (no error)=w736) -> (queue out=w744:refnum<queue>, # elements in queue=w745:i32)  [unwired: 1 in, 6 out]
            n366 = property class="Str"(reference=w749, error in=w736, "Value"="Flushing: Don't Panic. ") -> (reference out=w748:refnum<vi>, error out=w725:errorcluster)
            n367 = case "Batch Binning" shown="True" w737 {
              selector: w737 -> [_ w776]
              tunnel: w745 -> [_ w784]
              tunnel: w744 -> [w774 w783]
              tunnel: w743 -> [_ w782]
              tunnel: w742 -> [_ w781]
              tunnel: w741 -> [_ w780]
              tunnel: w740 -> [_ w779]
              tunnel: [w774 w778] -> w731
              tunnel: w738 -> [w772 w777]
              tunnel: [w773 w775] -> w735
              frame False {
                n368 = Array Size(array=w772) -> (size(s)=w773:i32)
              }
              frame True {
                n369 = for {
                  N: w784 -> [_]
                  shift-right: [w793] -> w778
                  shift-left: w783 -> [w799]
                  tunnel: w782 -> [w798]
                  tunnel: w781 -> [w797]
                  tunnel: w776 -> [w796]
                  tunnel: w780 -> [w795]
                  tunnel: w779 -> [w794]
                  tunnel: w777 -> [w788]
                  tunnel: [w785] -> w775
                  n370 = Dequeue Element(queue=w799) -> (queue out=w792:refnum<queue>, element=w791:T10)  [unwired: 2 in, 2 out]
                  n371 = Unbundle By Name(w791) -> ("Spectra"=w789:sgl[])
                  n372 = call "SpectrumBinning_NoGraph.vi"("XScale.Maximum"=w798, "BinType"=w794, "BinWidth"=w797, "Enable"=w796, "Signal"=w789, "m/z Array"=w788, "XScale.Minimum"=w795) -> ("Spectrum"=w787:dbl[], "m/z Array"=w786:dbl[])  [unwired: 2 in, 1 out]
                  n373 = Bundle By Name(cluster=w791, "Spectra"=w787) -> (w790:T10)
                  n374 = Array Size(array=w786) -> (size(s)=w785:i32)
                  n375 = Enqueue Element(queue=w792, element=w790) -> (queue out=w793:refnum<queue>)  [unwired: 2 in, 2 out]
                }
              }
            }
            n376 = Bundle By Name(cluster=w728, "File Header.SpecLength"=w735) -> ()  [unwired: 1 out]
            n377 = call "Flush(DepthProfiling_3D).vi"("data buffer in"=w731, "Image in"=w734, "Z Counter"=w732, "Image Params"=w728, "DepthProfileBuffer in"=w727, "Y_img"=w729, "error in"=w725, "conv. coeff."="conv. coeff.") -> ("Image out"=w733:dbl[][][], "DepthProfileBuffer out"=w726:T29, "error out"=w724:errorcluster)  [unwired: 4 in, 1 out]
            n378 = call <vilib>:"General Error Handler.vi"() -> ("error out"=w766:errorcluster)  [unwired: 11 in, 4 out]
            n379 = Increment(x=w729) -> (x+1=w760:i32)
            n380 = property class="Str"(reference=w748, error in=w724, "Value"="") -> ()  [unwired: 2 out]
            "Line#" <- w729
          }
          frame "ScanResult" {
            # "For comapatibility with other static subprogram, drive the loop going"
            n381 = Increment(x=w817) -> (x+1=w820:T3)
            n382 = Bundle By Name(cluster=w818, "State"=w820) -> (w821:T15)
            n383 = Enqueue Element(queue=w819, element=w821) -> ()  [unwired: 2 in, 3 out]
          }
          frame "CheckEndCondition" {
            w838 = 2  # axis:Z
            w845 = 1  # axis:Y
            # "Some bug may exist"
            # "fitted for 3D imaing, \nmay not fit for binary file conversion"
            # "Add condition:\nreader quit due to file ends"
            n384 = Unbundle By Name(w830) -> ("Scan#"=w836:i32, "File Header.Dimension"=w846:i32[])
            n385 = Index Array(array=w846, index #1=w845, index #2=w838) -> (element #1=w835:i32, element #2=w827:i32)
            n386 = Multiply(x=w835, y=w827) -> (x*y=w837:i32)
            n387 = Quotient & Remainder(x=w836, y=w835) -> (x-y*floor(x/y)=w828:i32, floor(x/y)=w826:i32)
            n388 = Subtract(x=w837, y=w836) -> (x-y=→"remaining lines":i32)
            n389 = Equal To 0? "2D_Image finished?"(x=w828) -> (x = 0?=w825:bool)
            n390 = Greater Or Equal? "3D_Image finished"(x=w826, y=w827) -> (x >= y?=w824:bool)
            n391 = case "One Image Finish" shown="True" w825 {
              tunnel: w826 -> [_ w850]
              tunnel: [T15 {"State"=enum."PrepScanParams", "Para."=variant} w860] -> w833
              tunnel: w832 -> [w848 w866]
              tunnel: [w848 w865] -> w831
              tunnel: w829 -> [_ w863]
              frame False {
                # "Continue next line scan"
              }
              frame True {
                # "If the file exist, error will be thrown out \nand will crash the expt !, proper error handling needed"
                # "to be done"
                # "A signal image finished in 3D imaging."
                n392 = Unbundle By Name(w863) -> ("file path"=w861:path)
                n393 = Enqueue Element(queue=w866, element=T15 {"State"=enum."Close", "Para."=variant}) -> (queue out=w865:refnum<queue>)  [unwired: 2 in, 2 out]
                n394 = Strip Path(path=w861) -> (stripped path=w862:path, name=w851:string)
                n395 = Format Value(string ("")="_", format string="%04d", value (0)=w850) -> (output string=w856:string)
                n396 = xnode "Match Regular Expression"("input string"=w851, "regular expression"="((_[0-9]+)?)(\\..[^.]*$)") -> ("before match"=w858:string, "submatch 3"=w853:string)  [unwired: 4 in, 6 out]
                n397 = Concatenate Strings "Append depth number"(w858, w856, w853) -> (w852:string)
                n398 = Build Path(base path=w862, name or relative path=w852) -> (appended path=w859:path)
                n399 = Bundle By Name(cluster=T15 {"State"=enum."Open", "Para."=variant}, "Para."=w859) -> (w860:T15)
              }
            }
            n400 = Select(t=T15 {"State"=enum."Close", "Para."=variant}, s=w824, f=w833) -> (s? t:f=w839:T15)
            n401 = Enqueue Element(queue=w831, element=w839) -> ()  [unwired: 2 in, 3 out]
          }
          frame "Close" {
            # "need to reset registers?\n\nNo"
            n402 = Unbundle By Name(w990) -> ("file refnum"=w991:refnum<file>)
            n403 = Close File(refnum=w991, error in=w988) -> (error out=w987:errorcluster)  [unwired: 1 out]
            n404 = call <vilib>:"Clear Errors.vi"("error in (no error)"=w987) -> ()  [unwired: 6 in, 1 out]
            n405 = Unbundle By Name(w1004) -> ("ControlRefs.ProcCore_CtrlQueue"=w999:refnum<queue>, "ControlRefs.WriterSIG"=w1003:refnum<queue>)
            n406 = property on="Cancel" class="Bool"("Visible"=FALSE) -> ()  [unwired: 2 in, 2 out]
            n407 = property on="Close/Quit" class="Bool (strict)"("BoolText.Text"="Done" ("Boolean Text.Text")) -> ()  [unwired: 2 in, 2 out]
            n408 = Bundle By Name(cluster=T23 {"Command"=enum."SetWriterRef", "Params"=variant} ("element"), "Command"=ProcessStates."StopSave") -> (w998:T23)
            n409 = Bundle By Name(cluster=T23 {"Command"=enum."SetWriterRef", "Params"=variant} ("element"), "Command"=ProcessStates."SetWriterRef", "Params"=w1003) -> (w1006:T23)
            n410 = Enqueue Element(queue=w999, element=w998) -> (queue out=w997:refnum<queue>, error out=w996:errorcluster)  [unwired: 2 in, 1 out]
            n411 = Enqueue Element(queue=w997, element=w1006, error in (no error)=w996) -> (error out=w995:errorcluster)  [unwired: 1 in, 2 out]
            n412 = call <vilib>:"Clear Errors.vi"("error in (no error)"=w995) -> ()  [unwired: 6 in, 1 out]
          }
          frame "Quit" {
            n413 = disable-structure shown="Enabled" {
              disable-tunnel: w1015 -> [w1029 _]
              frame Enabled {
                # "maybe not needed anymore, needed to be tested!!"
                # "Bad solution: have upper level jump out wait queue"
                n414 = Enqueue Element(queue=w1029, element=T26 {"Line Start"=[], "Line End"=[], "HighSpeed"=0.0, "ScanSpeed"=0.0, "KeepStill(ms)"=0, "InstruParams"=[]}) -> (error out=w1027:errorcluster)  [unwired: 2 in, 2 out]
                n415 = call <vilib>:"Clear Errors.vi"("error in (no error)"=w1027) -> ()  [unwired: 6 in, 1 out]
              }
              frame Disabled {
              }
            }
            n416 = Release Queue(queue=w1023, error in (no error)=w1010) -> (error out=w1012:errorcluster)  [unwired: 1 in, 2 out]
            n417 = Generate User Event(user event=w1020, event data cluster=cluster{bool} {TRUE} ("event data")) -> (user event out=w1018:refnum<user-event>, error out=w1017:errorcluster)  [unwired: 2 in]
            n418 = Destroy User Event(user event=w1018, error in=w1017) -> (error out=w1016:errorcluster)
            n419 = Merge Errors(w1016, w1012) -> (w1011:errorcluster)
          }
          frame "Refresh_Image" {
            w1043 = 0.0 ("Z Scale.Range:Minimum")
            # "Call command has to be push to the end not start of the queue."
            n420 = Unbundle By Name(w1048) -> ("Para."=w1047:variant)
            n421 = Variant To Data(type=1 ("PeakOI #"), Variant=w1047) -> (data=w1044:i32)  [unwired: 1 in, 1 out]
            n422 = Array Subset(array=w1051, index (dim 2)=w1044, length (dim 2)=1 ("length")) -> (w1050:dbl[][][])  [unwired: 4 in]
            n423 = control-ref of="ImagePreview"() -> (w1032:refnum<vi>)
            n424 = Array Size(array=w1050) -> (size(s)=w1049:i32[])
            n425 = Index Array(array=w1049) -> (element #1=w1042:i32, element #2=w1041:i32)  [unwired: 3 in, 1 out]
            n426 = Max & Min(x=w1042, y=w1041) -> (max(x,y)=w1040:i32)  [unwired: 1 out]
            n427 = Reshape Array(w1050, w1042, w1041) -> (w1031:dbl[][])
            n428 = property on="Fix race condition \n(autoscale related)" class="IntGraph (strict)"(reference=w1032, "Value"=w1031) -> (reference out=w1033:refnum<vi>, error out=w1034:errorcluster)  [unwired: 1 in]
            n429 = property class="IntGraph (strict)"(reference=w1033, error in=w1034) -> (reference out=w1039:refnum<vi>, "ZScale.Maximum"=w1036:dbl)  [unwired: 1 out]
            n430 = Array Max & Min(array=w1031) -> (max value=w1038:dbl)  [unwired: 3 out]
            n431 = Select(t=w1038, s="AutoScaleZ", f=w1036) -> (s? t:f=w1037:dbl)
            n432 = property class="IntGraph (strict)"(reference=w1039, "ZScale.Maximum"=w1037, "ZScale.Minimum"=w1043, "XScale.Minimum"=w1043, "XScale.Maximum"=w1040, "YScale.Minimum"=w1043, "YScale.Maximum"=w1040) -> ()  [unwired: 1 in, 2 out]
          }
          frame "Refresh_Profile" {
            n433 = Unbundle By Name(w1059) -> ("mzArray"=w1058:dbl[])
            n434 = Subtract(x="m/z (Da)", y="Integration Width (±Da)") -> (x-y=w1065:dbl)
            n435 = Add(x="m/z (Da)", y="Integration Width (±Da)") -> (x+y=w1064:dbl)
            n436 = Threshold 1D Array(2:w1065, 3:w1058) -> (0:w1068:dbl)  [unwired: 1 in]
            n437 = Round Toward -Infinity(1:w1068) -> (0:w1066:dbl)
            n438 = Threshold 1D Array(1:w1066, 2:w1064, 3:w1058) -> (0:w1067:dbl)
            n439 = for {
              tunnel: w1061 -> [w1081] mode=indexing
              tunnel: [w1077] -> w1060 mode=indexing
              tunnel: w1067 -> [w1076]
              tunnel: w1066 -> [w1075]
              n440 = Unbundle By Name(w1081) -> ("Spectra"=w1080:sgl[])
              n441 = Subtract(x=w1076, y=w1075) -> (x-y=w1079:dbl)
              n442 = Array Subset(array=w1080, index=w1075, length=w1079) -> (w1078:sgl[])
              n443 = call-poly <vilib>:"Mean.vi"("X"=w1078) -> ("mean"=w1077:dbl)  [unwired: 1 out]
            }
            "Depth Profile" <- w1060
          }
          frame "Refresh_Spectra" {
            n444 = Decrement(x="Shot#") -> (x-1=w1091:i32)
            n445 = for {
              N: "#Layers" -> [_]
              tunnel: w1089 -> [w1111]
              tunnel: w1091 -> [w1109]
              shift-right: [w1107] -> w1095
              shift-left: _ -> [w1106]
              tunnel: [w1104] -> w1093
              tunnel: [w1103] -> _ mode=indexing
              i -> [w1104]
              n446 = Add(x=w1109, y=w1104) -> (x+y=w1108:i32)
              n447 = Index Array(array=w1111, index=w1108) -> (element=w1110:T10)
              n448 = Unbundle By Name(w1110) -> ("Spectra"=w1103:sgl[])
              n449 = Equal To 0?(x=w1104) -> (x = 0?=w1105:bool)
              n450 = case shown="False" w1105 {
                tunnel: [w1114 w1115] -> w1107
                tunnel: w1106 -> [w1113 _]
                tunnel: w1103 -> [w1112 w1115]
                frame False {
                  n451 = Add(x=w1112, y=w1113) -> (x+y=w1114:sgl[])
                }
                frame True {
                }
              }
            }
            n452 = Unbundle By Name(w1088) -> ("mzArray"=w1096:dbl[])
            n453 = Increment(x=w1093) -> (x+1=w1092:i32)
            n454 = Reciprocal(x=w1092) -> (1/x=w1094:dbl)
            n455 = control-ref of="Spectra"() -> (w1084:refnum<vi>)
            n456 = Multiply(x=w1095, y=w1094) -> (x*y=w1090:dbl[])
            n457 = call-poly "SpecBinning.vi"("BinType"="BinType", "BinWidth"="BinWidth", "Signal"=w1090, "m/z Array"=w1096, "GraphRef."=w1084) -> ("BinnedSpectrum"=→"Spectra":cluster{"m/z Array":dbl[], "Signal":dbl[]})  [unwired: 5 in, 1 out]
          }
          frame "SaveMiddleFile" {
            n458 = call <vilib>:"Dflt Data Dir.vi"() -> ("App:Default Data Directory"=w1127:path)
            n459 = feedback #13(w1127) -> (w1125:path)
            n460 = Strip Path(path=w1125) -> (stripped path=w1121:path, name=w1122:string)
            n461 = call "File Dialog"("start path"=w1121, "default name"=w1122, "pattern (all files)"="*.dp.bin", "pattern label"="Depth Profile File") -> ("selected path"=w1123:path, "cancelled"=w1118:bool, "error out"=w1126:errorcluster)  [unwired: 8 in, 1 out]
            n462 = case shown="False" w1118 {
              tunnel: w1123 -> [w1138 _]
              tunnel: [w1138 w1139] -> w1124
              tunnel: w1125 -> [_ w1139]
              tunnel: w1126 -> [w1137 _]
              tunnel: w1116 -> [w1134 _]
              tunnel: [w1136 _] -> _
              tunnel: w1117 -> [w1135 _]
              frame False {
                n463 = call "DepthProfileFormat_Writer.vi"("error in"=w1137, "DepthProfilingArray"=w1134, "AcquisitionParams."=w1135, "depth profile file path"=w1138) -> ("error out"=w1136:errorcluster)  [unwired: 7 in]
              }
              frame True {
              }
            }
            n464 = feedback-in #13(w1124) -> ()
          }
          frame "Save_Image" {
            # "Call command has to be push to the end not start of the queue."
            n465 = control-ref of="Peaks of Interest"() -> (w1151:refnum<vi>)
            n466 = Unbundle By Name(w1182) -> ("Para."=w1181:variant)
            n467 = property class="Tbl (strict)"(reference=w1151) -> ("Value"=w1150:string[][])  [unwired: 1 in, 2 out]
            n468 = Variant To Data(type=1 ("PeakOI #"), Variant=w1181) -> (data=w1149:i32)  [unwired: 1 in, 1 out]
            n469 = Unbundle By Name(w1142) -> ("file path"=w1141:path)
            n470 = Index Array(array=w1150, index (row) #1=w1149, index (col) #1=0 ("disabled index (col)"), index (row) #2=w1149, index (col) #2=1 ("disabled index (col)")) -> (element #1=w1146:string, element #2=w1145:string)
            n471 = control-ref of="ImagePreview"() -> (w1176:refnum<vi>)
            n472 = Strip Path(path=w1141) -> (stripped path=w1156:path, name=w1160:string)
            n473 = Array Subset(array=w1185, index (dim 2)=w1149, length (dim 2)=1 ("length")) -> (w1184:dbl[][][])  [unwired: 4 in]
            n474 = property class="IntGraph (strict)" props=["Color Table", "ZScale", "Maximum", "ZScale", "Minimum", "XScale", "Minimum", "XScale", "Maximum", "YScale", "Minimum", "YScale", "Maximum"](reference=w1176) -> ("Color Table"=w1153:u32[], "ZScale.Maximum"=w1154:dbl, "ZScale.Minimum"=w1155:dbl)  [unwired: 1 in, 6 out]
            n475 = xnode "Match Regular Expression"("input string"=w1160, "regular expression"="(\\..[^.]*$)") -> ("before match"=w1173:string)  [unwired: 4 in, 4 out]
            n476 = Format Into String(format string="_%s(+-%s)", w1146, w1145) -> (resulting string=w1172:string)  [unwired: 2 in, 1 out]
            n477 = Array Size(array=w1184) -> (size(s)=w1183:i32[])
            n478 = Index Array(array=w1183) -> (element #1=w1178:i32, element #2=w1177:i32)  [unwired: 3 in, 1 out]
            n479 = Concatenate Strings(w1173, w1172, ".png" ("string")) -> (w1157:string)
            n480 = Reshape Array(w1184, w1178, w1177) -> (w1152:dbl[][])
            n481 = Subtract(x=w1154, y=w1155) -> (x-y=w1166:dbl)
            n482 = Build Path(base path=w1156, name or relative path=w1157) -> (appended path=w1158:path)
            n483 = Subtract(x=w1152, y=w1155) -> (x-y=w1175:dbl[][])
            n484 = Divide(x=256.0 ("Img_coeff."), y=w1166) -> (x/y=w1168:dbl)
            n485 = Array Size(array=w1175) -> (size(s)=w1161:i32[])
            n486 = Compound Arithmetic op=MULTIPLY(w1168, w1175) -> (w1169:dbl[][])
            n487 = Transpose 2D Array(2D array=w1169) -> (transposed array=w1170:dbl[][])
            n488 = Index Array(array=w1161) -> (element #1=w1163:i32, element #2=w1164:i32)  [unwired: 2 in]
            n489 = Round Toward -Infinity(1:w1170) -> (0:w1171:dbl[][])
            n490 = Multiply(x=w1163, y=w1164) -> (x*y=w1165:i32)
            n491 = To Unsigned Byte Integer(number=w1171) -> (unsigned 8bit integer=w1162:u8[][])
            n492 = disable-structure shown="Enabled" {
              disable-tunnel: w1153 -> [w1201 _]
              disable-tunnel: w1158 -> [w1200 w1204]
              disable-tunnel: w1162 -> [w1196 w1205]
              disable-tunnel: w1163 -> [w1194 _]
              disable-tunnel: w1164 -> [w1193 _]
              disable-tunnel: w1165 -> [w1192 _]
              frame Enabled {
                n493 = Reshape Array(w1196, w1192) -> (w1195:u8[])
                n494 = Bundle By Name(cluster=T27 {"image type"=0, "image depth"=32, "image"=[], "mask"=[], "colors"=[], "Rectangle"={"left"=0, "top"=0, "right"=256, "bottom"=256}} ("Image Data 2"), "colors"=w1201, "image type"=0, "image depth"=8, "image"=w1195, "Rectangle.right"=w1194, "Rectangle.bottom"=w1193) -> (w1191:T27)
                n495 = call <vilib>:"Write PNG File.vi"("image data"=w1191, "path to PNG file"=w1200) -> ("error out"=w1190:errorcluster)  [unwired: 8 in, 1 out]
                n496 = call <vilib>:"Clear Errors.vi"("error in (no error)"=w1190) -> ()  [unwired: 6 in, 1 out]
              }
              frame Disabled {
                n497 = call "IMAQ ArrayToImage"("Image Pixels (U8)"=w1205) -> ("Image Out"=w1203:T30)  [unwired: 9 in, 1 out]
                n498 = call-poly "IMAQ Write File 2"("TIFF Options"=T28 {"Rows Per Strip"=0, "Photometric"=1, "Compression Type"=3}, "File Path"=w1204, "Image"=w1203) -> ()  [unwired: 7 in, 2 out]
              }
            }
          }
          frame "SetPeakOI" {
            n499 = Unbundle By Name(w1325) -> ("PeakOI"=w1321:cluster{"m/z":dbl, "Width(+/-)":dbl}[])
            n500 = Unbundle By Name(w1327) -> ("Para."=w1326:variant)
            n501 = Variant To Data(type=w1321, Variant=w1326) -> (data=w1323:cluster{"m/z":dbl, "Width(+/-)":dbl}[], error out=w1324:errorcluster)  [unwired: 1 in]
            n502 = Select(t=w1321, s=w1324, f=w1323) -> (s? t:f=w1322:cluster{"m/z":dbl, "Width(+/-)":dbl}[])
            n503 = Bundle By Name(cluster=w1325, "PeakOI"=w1322) -> (w1330:T11)
          }
          frame Default {
          }
        }
        n504 = call <userlib>:"ErrorLog.vi"("error in (no error)"=w376) -> ("error out"=w375:errorcluster)  [unwired: 10 in]
      }
      frame Error {
      }
    }
    "Iteration" <- w349
  }
  n505 = Release Queue "Release Queue\nAfter all quit."(queue=w20, error in (no error)=w22) -> (error out=→"error out":errorcluster)  [unwired: 1 in, 2 out]
  n506 = disable-structure "For legacy files, manually add EOL mark" shown="Disabled" {
    frame Disabled {
      w1350 = FALSE  # True for missing EOL (Legacy)
      n507 = And(y=w1350) -> (x .and. y?=w1349:bool)  [unwired: 1 in]
      n508 = case "For Legacy Code" shown="True" w1349 {
        tunnel: _ -> [_ w1356]
        frame False {
        }
        frame True {
          n509 = Type Cast(type="", x=ProcessStates."EndOfLine") -> (*(type *) &x=w1355:string)
          n510 = Bundle By Name(cluster=T24 {"SampleRate"=-1.0, "TrigDelay"=0.0, "SpecLength"=0.0, "DAQ_Range"=0.0, "Average#"=0, "Position"=[], "Spectrum"=[], "Calibr."=[], "Pressure"=-1.0, "Desp_LaserEnergy"=-1.0, "PI_LaserEnergy"=-1.0, "Voltages Table"=[], "ProcMode"=enum."None", "Threshold"=-1.0, "Comment"="", "TickCount"=0.0, "Time Stamp"=timestamp(0 s since 1904-01-01)} ("Value"), "Comment"=w1355) -> (w1351:T24)
          n511 = Enqueue Element At Opposite End(queue=w1356, element=w1351) -> ()  [unwired: 2 in, 3 out]
        }
      }
    }
    frame Enabled {
    }
  }
